vi "Machine_Etat_M1.vi"() -> ()   [LabVIEW 2017]
uses:
  Commande 1.ctl
  enum_tour.ctl
  <vilib>/Platform/TimedLoop/XDataNode/timing_clust.ctl
  <vilib>/Platform/TimedLoop/XDataNode/nitl_modes.ctl
  <vilib>/Platform/TimedLoop/XDataNode/wakeup.ctl
  enum_bras.ctl
  <vilib>/myRIO/Instrument Drivers/Onboard IO/DIO/typedefs/DIO Reference.ctl
  <vilib>/myRIO/Common/Instrument Driver Framework/Utilities/typedefs/myRIO Generic Hardware Reference.ctl
  <vilib>/myRIO/Common/Instrument Driver Framework/Utilities/typedefs/Hardware Version Enum.ctl
  <vilib>/myRIO/Common/Instrument Driver Framework/Utilities/typedefs/myRIO v1.0 Reference.ctl
  <vilib>/myRIO/Common/Instrument Driver Framework/Utilities/typedefs/Generic FPGA Reference.ctl
  <vilib>/myRIO/Common/Instrument Driver Framework/myRIO v1.0/DIO/typedefs/DIO Channels List.ctl
  <vilib>/myRIO/Common/Instrument Driver Framework/myRIO v1.0/DIO/typedefs/DIO Channels Enum.ctl
  <vilib>/userdefined/High Color/nirio_resource_hc.ctl
  <vilib>/myRIO/Common/Instrument Driver Framework/Utilities/vis/Is FPGA Ref Available.vi
  <vilib>/myRIO/Common/Instrument Driver Framework/myRIO v1.0/DIO/vis/myRIO v1.1 Open DIO.vi
  <vilib>/myRIO/Instrument Drivers/Onboard IO/DIO/vis/Write.vi
  <vilib>/myRIO/Common/Instrument Driver Framework/Utilities/vis/Validate Channels.vi
  <vilib>/myRIO/Common/Instrument Driver Framework/myRIO v1.0/DIO/vis/myRIO v1.0 Reserve DIO.vi
  <vilib>/myRIO/Common/Instrument Driver Framework/myRIO v1.0/Resource Manager/vis/myRIO v1.0 Reserve Channel List.vi
  <vilib>/myRIO/Common/Instrument Driver Framework/myRIO v1.0/DIO/vis/myRIO v1.0 Build MUX Configuration DIO.vi
  <vilib>/myRIO/Common/Instrument Driver Framework/myRIO v1.0/Resource Manager/vis/myRIO v1.0 Reserve Channel.vi
  <vilib>/myRIO/Common/Instrument Driver Framework/myRIO v1.0/Resource Manager/vis/myRIO v1.0 Unreserve Channel.vi
  <vilib>/myRIO/Common/Instrument Driver Framework/myRIO v1.0/Resource Manager/vis/myRIO v1.0 Create Configuration List.vi
  <vilib>/myRIO/Common/Instrument Driver Framework/myRIO v1.0/Resource Manager/vis/myRIO v1.0 Build Mutex Name.vi
  <vilib>/Utility/VariantDataType/GetNumericInfo.vi
  <vilib>/Utility/error.llb/Error Cluster From Error Code.vi
  <vilib>/myRIO/Common/Instrument Driver Framework/myRIO v1.0/myRIO v1.1 Open.vi
  <vilib>/myRIO/Common/Instrument Driver Framework/Utilities/vis/IO Manager.vi
  <vilib>/myRIO/Common/Instrument Driver Framework/Utilities/vis/Configuration Manager.vi
  <vilib>/myRIO/Common/Instrument Driver Framework/myRIO v1.0/Resource Manager/vis/myRIO v1.0 Configure IO.vi
  <vilib>/myRIO/Common/Instrument Driver Framework/myRIO v1.0/myRIO v1.0 Close.vi
  <vilib>/myRIO/Common/Instrument Driver Framework/myRIO v1.0/DIO/vis/myRIO v1.0 Write DIO.vi
  <vilib>/Platform/TimedLoop/XDataNode/XDataNode.xnode
  <vilib>/myRIO/Express VI/Onboard Devices/LED/LED Express VI.xnode
  <vilib>/myRIO/Instrument Drivers/Onboard IO/DIO/vis/myRIO DIO Open.xnode
  <vilib>/Platform/TimedLoop/XDataNode/XDNodeRunTimeDep.lvlib
  <vilib>/myRIO/Instrument Drivers/Onboard IO/DIO/DIO.lvlib
panel:
  out "Vert : dévi à droite 2":bool
  out "Graphe déroulant 2":u32(graph)
  out "x > y ? 2":bool[](array[boolean])
  out "Cluster 3":T1
  out "4 LED droite 2":bool[](array[boolean])
  out "4 LED gauche 2":bool[](array[boolean])
  out "droite 2":u32
  out "gauche\n 2":u32
  out "Énum 2":T2
  out "seuil":u32
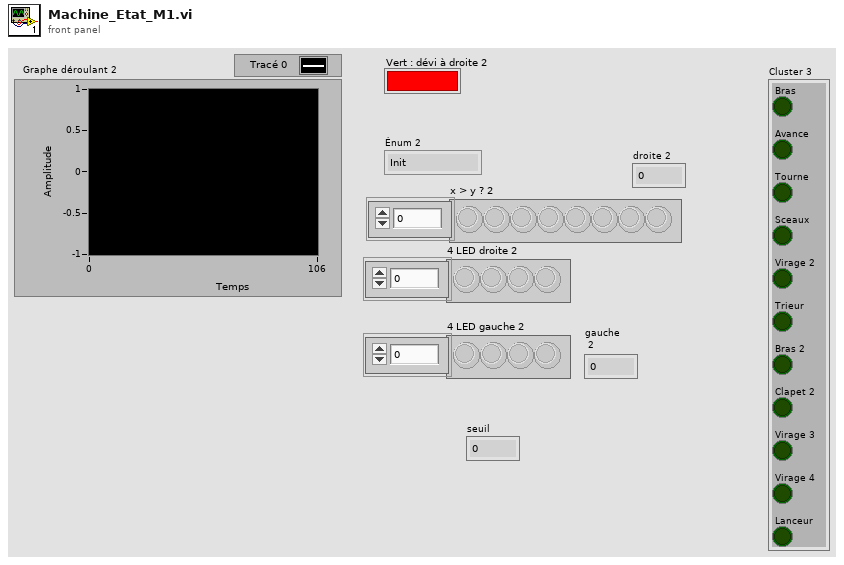
[diagram p1: front panel]
types:
  T1 = typedef "Voyant machine d'état.ctl" = cluster{"Bras":bool, "Avance":bool, "Tourne":bool, "Sceaux":bool, "Virage 2":bool, "Trieur":bool, "Bras 2":bool, "Clapet 2":bool, "Virage 3":bool, "Virage 4":bool, "Lanceur":bool}
  T2 = typedef "Commande 1.ctl" = enum16{"Init", "Bras", "Clapet 1", "Monter_bras", "Virage 1", "Sceaux 0", "Sceaux 1", "Sceaux 2", "Sceaux 3", "Sceaux 4", "Virage 2", "Recule", "Trieur", "Bras 2", "Intersection", "Clapet 2", "Virage 3", "Virage 4", "Avance", "Lanceur", "End", "Monter_bras1", "Monter_bras2", "Avance1", "Avance2", "Intersection1", "Avance3", "Demi_tour", "Virage 5", "Virage 6", "Intersection2", "Intersection3", "Intersection4"}
  T3 = typedef "enum_tour.ctl" = enum16{"Tour1", "Tour2", "Tour3"}
  T4 = typedef "XDNodeRunTimeDep.lvlib/timing_clust.ctl" = cluster{"Expected End [f-1]":u64, "Actual End [f-1]":u64, "Finished Late? [f-1]":bool, "Expected End [i-1]":u64, "Actual End [i-1]":u64, "Finished Late? [i-1]":bool, "Expected Start [i]":u64, "Actual Start [i]":u64, "Expected Start [f]":u64, "Actual Start [f]":u64, "Source Name":string, "Structure Name":string, "Period":i64, "Deadline":i64, "Offset":i64, "Start":i64, "Priority":i32, "Timeout":i32, "Mode":T5, "Wakeup Reason":T6, "Error":errorcluster, "Source Type":string, "Secondary Source Type":string, "Global End Time":u64, "Global Start Time":u64, "Frame Duration":u64, "Iteration Duration":u64, "Assigned CPU":i32, "I/O Scan Engine Mode":u32}
  T5 = typedef "XDNodeRunTimeDep.lvlib/nitl_modes.ctl" = enum32{"No Change", "Process missed periods, maintain original phase", "Discard missed periods, maintain original phase", "Process missed periods, ignore original phase", "Discard missed periods, ignore original phase"}
  T6 = typedef "XDNodeRunTimeDep.lvlib/wakeup.ctl" = enum32{"Normal", "Aborted", "Asynchronous wakeup", "Timing source error", "Timed loop error", "Timeout"}
  T7 = typedef "enum_bras.ctl" = enum16{"Depart Bras", "Clapet Bras", "Inactif Bras", "Seaux Bras"}
  T8 = typedef "DIO.lvlib/DIO Reference.ctl" = cluster{"myRIO Reference":T9, "DIO Channels List":T13}
  T9 = typedef "myRIO Generic Hardware Reference.ctl" = cluster{"myRIO Model":T10, "myRIO Hardware Reference":T11}
  T10 = typedef "Hardware Version Enum.ctl" = enum16{"Unknown", "myRIO-1900", "myRIO-1950", "roboRIO", "NI ELVIS RIO CM"}
  T11 = typedef "myRIO v1.0 Reference.ctl" = cluster{"Generic FPGA Reference":T12, "Allow multiple opens":bool}
  T12 = typedef "Generic FPGA Reference.ctl" = refnum<k20>
  T13 = typedef "DIO Channels List.ctl" = T14[]
  T14 = typedef "DIO Channels Enum.ctl" = enum16{"Not Connected", "C/DIO0", "C/DIO1", "C/DIO2", "C/DIO3", "C/DIO4", "C/DIO5", "C/DIO6", "C/DIO7", "A/DIO0", "A/DIO1", "A/DIO2", "A/DIO3", "A/DIO4", "A/DIO5", "A/DIO6", "A/DIO7", "A/DIO8", "A/DIO9", "A/DIO10", "A/DIO11", "A/DIO12", "A/DIO13", "A/DIO14", "A/DIO15", "B/DIO0", "B/DIO1", "B/DIO2", "B/DIO3", "B/DIO4", "B/DIO5", "B/DIO6", "B/DIO7", "B/DIO8", "B/DIO9", "B/DIO10", "B/DIO11", "B/DIO12", "B/DIO13", "B/DIO14", "B/DIO15", "LED0", "LED1", "LED2", "LED3", "Button0", "DIO/DIO0", "DIO/DIO1", "DIO/DIO2", "DIO/DIO3", "DIO/DIO4", "DIO/DIO5", "DIO/DIO6", "DIO/DIO7", "DIO/DIO8", "DIO/DIO9", "SPI/CS0", "SPI/CS1", "SPI/CS2", "SPI/CS3", "LED RADIO (Green)", "LED RADIO (Red)", "LED COMM (Green)", "LED COMM (Red)", "LED MODE (Green)", "LED MODE (Red)"}
  T15 = typedef "nirio_resource_hc.ctl" = tag
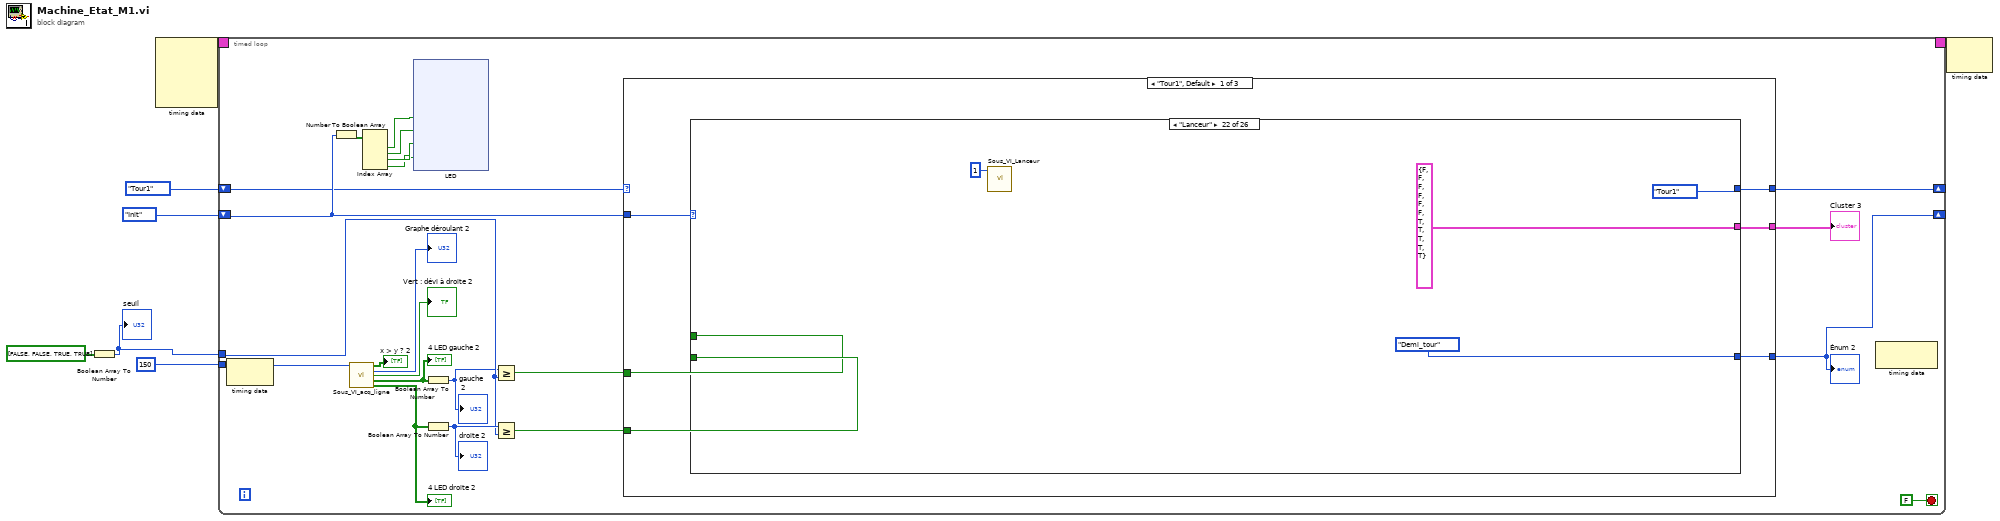
[diagram p0: block diagram]
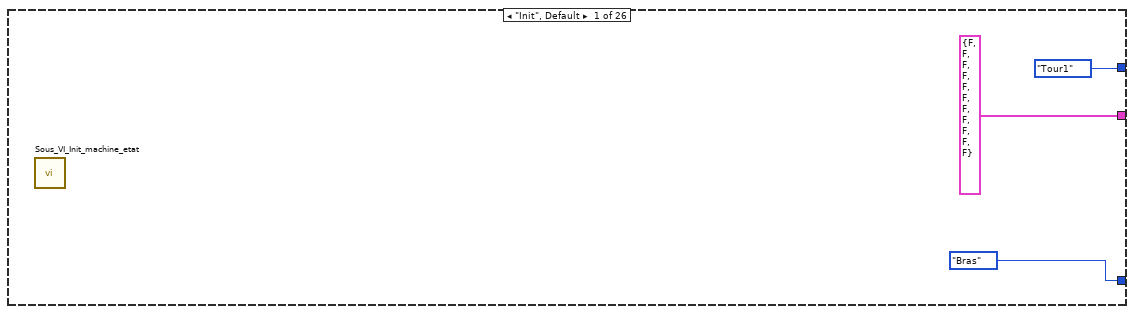
[diagram p2: hidden frame]
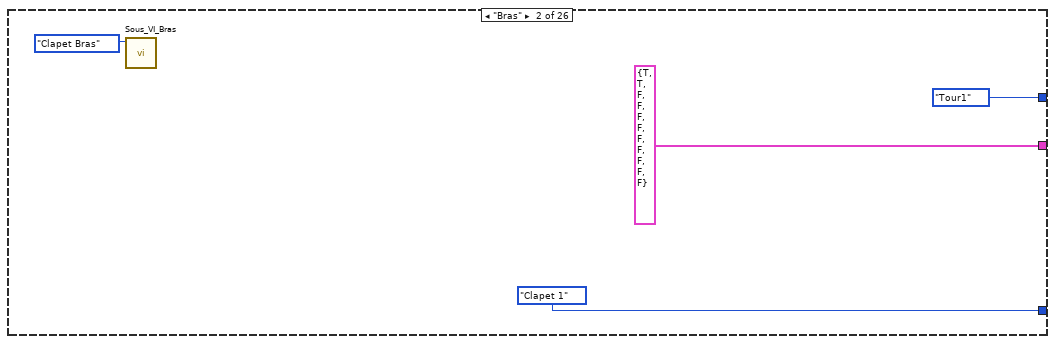
[diagram p3: hidden frame]
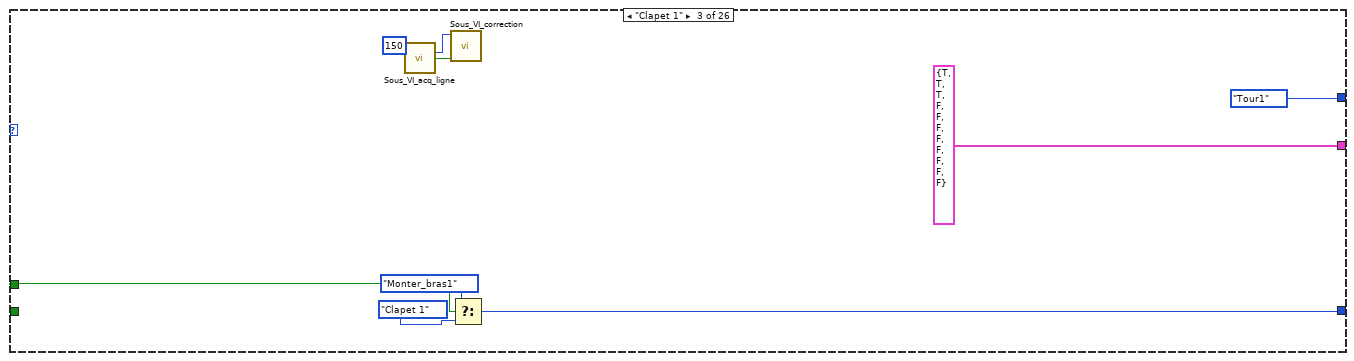
[diagram p4: hidden frame]
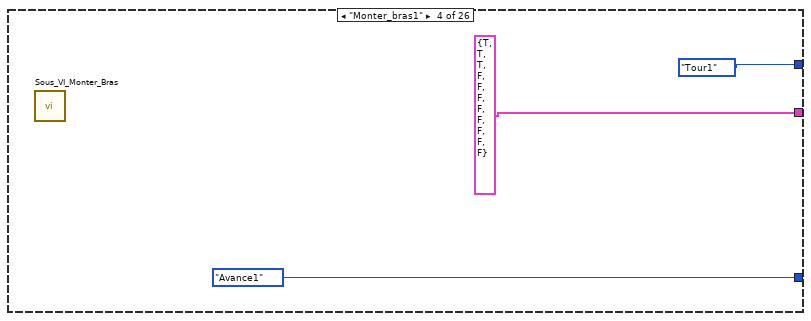
[diagram p5: hidden frame]
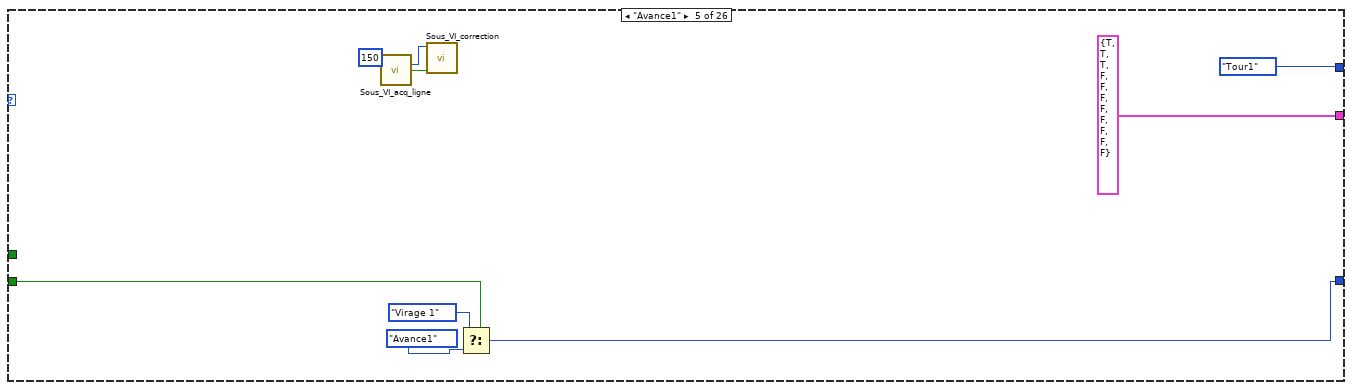
[diagram p6: hidden frame]
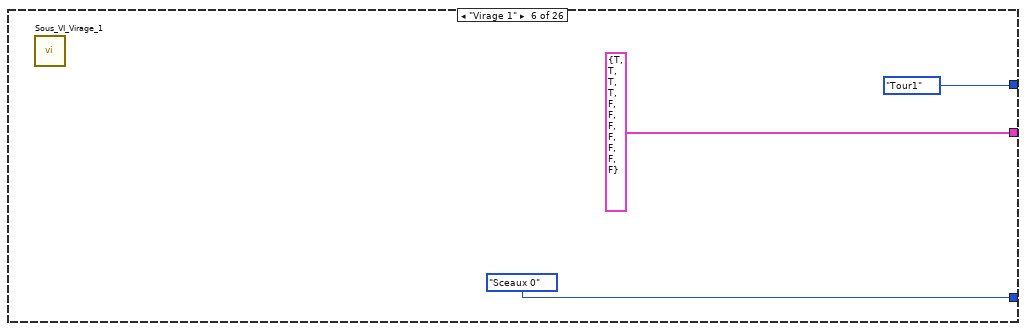
[diagram p7: hidden frame]
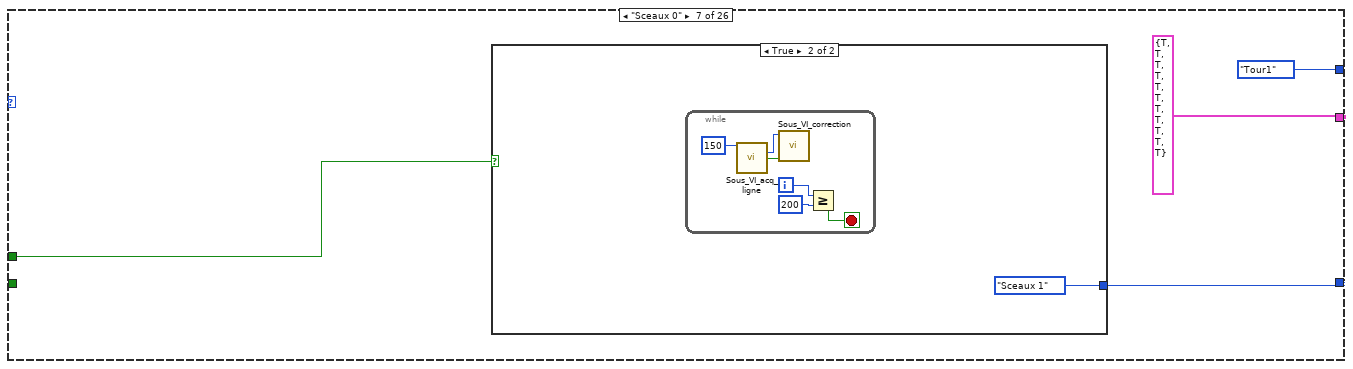
[diagram p8: hidden frame]
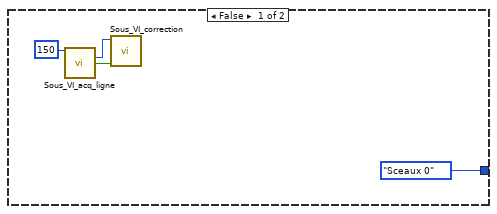
[diagram p9: hidden frame]
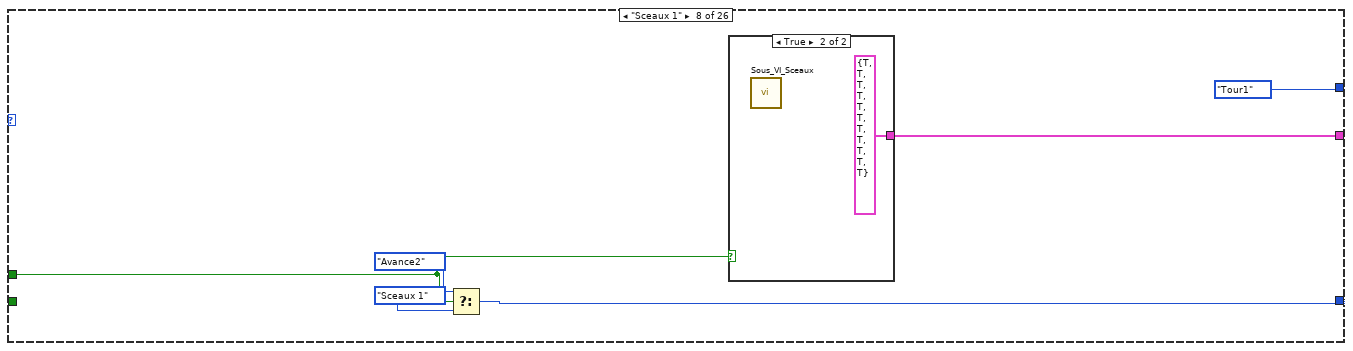
[diagram p10: hidden frame]
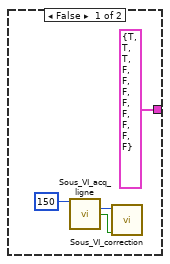
[diagram p11: hidden frame]
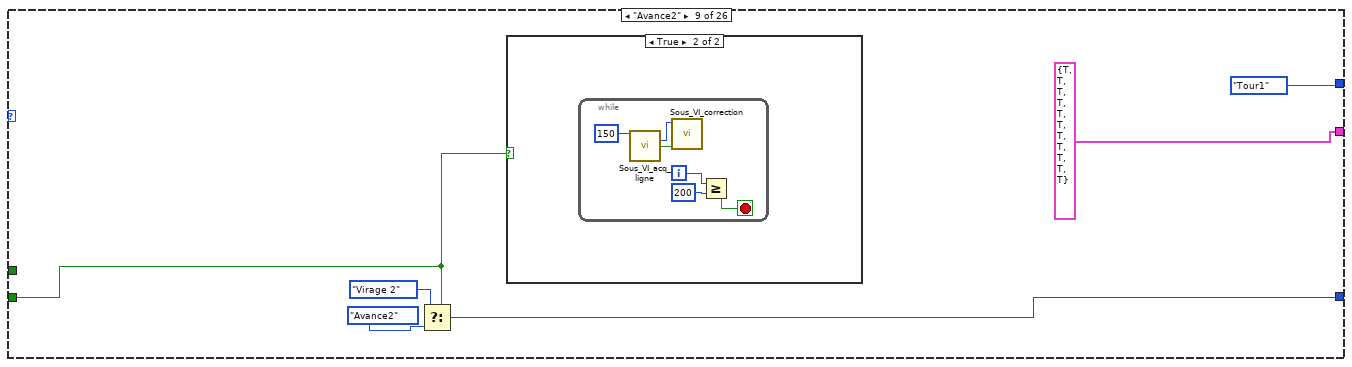
[diagram p12: hidden frame]
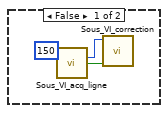
[diagram p13: hidden frame]
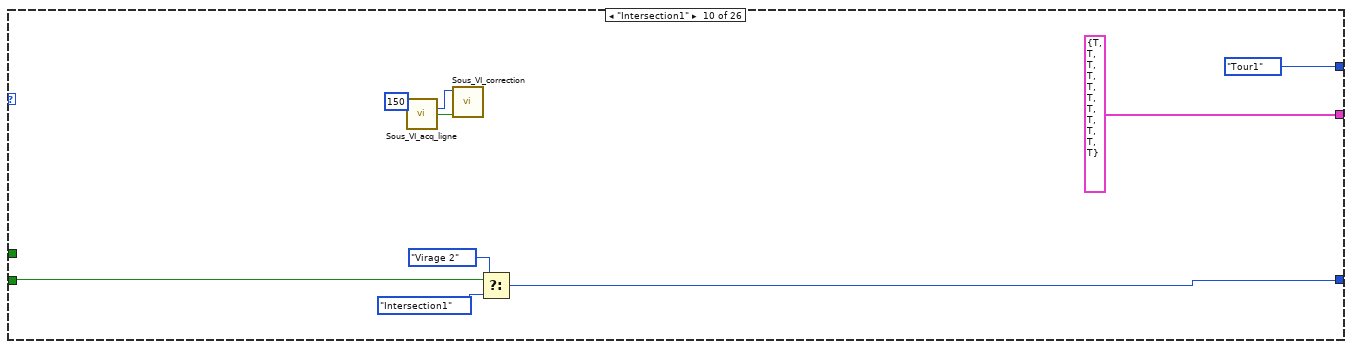
[diagram p14: hidden frame]
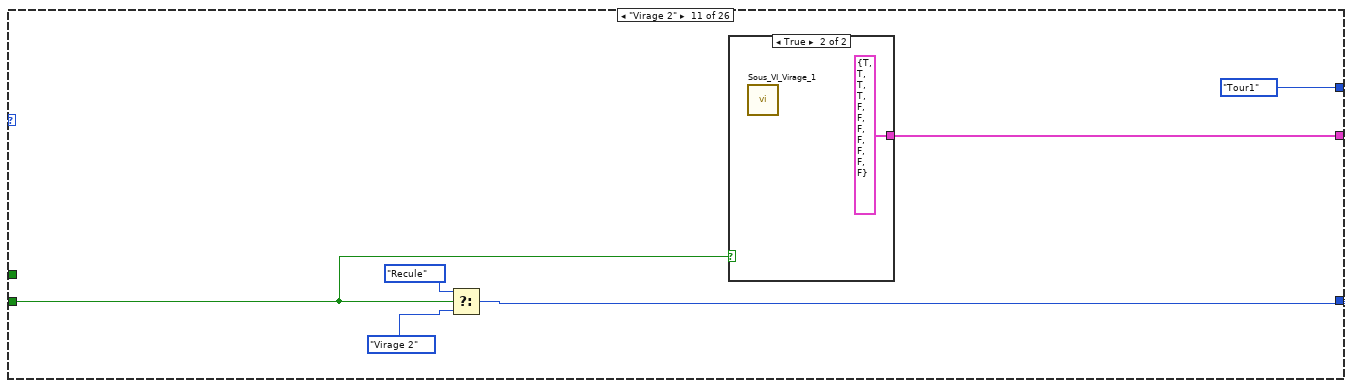
[diagram p15: hidden frame]
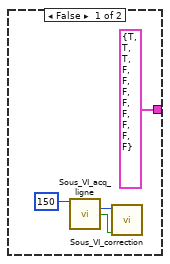
[diagram p16: hidden frame]
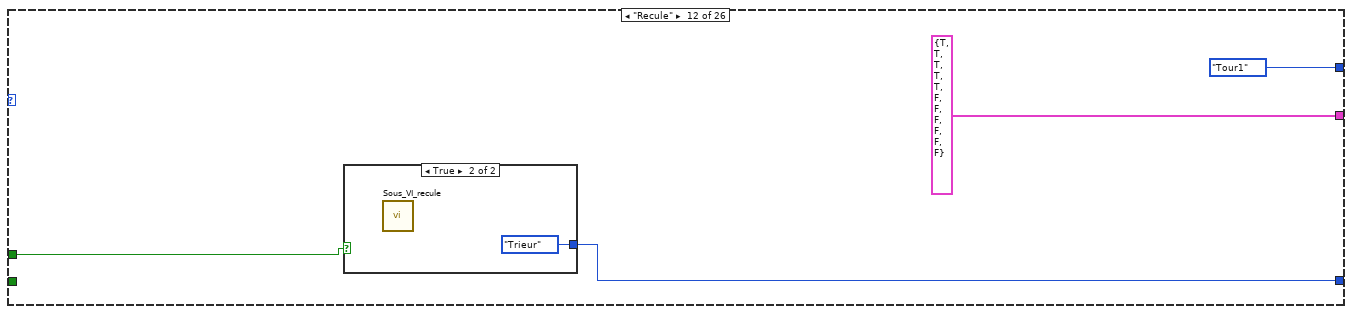
[diagram p17: hidden frame]
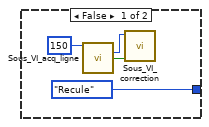
[diagram p18: hidden frame]
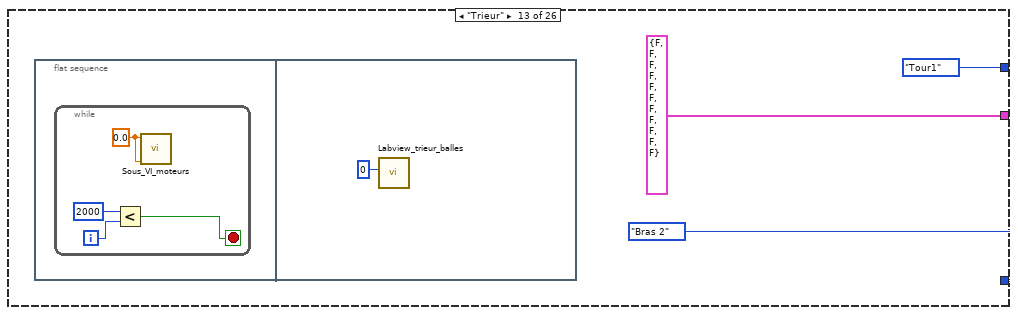
[diagram p19: hidden frame]
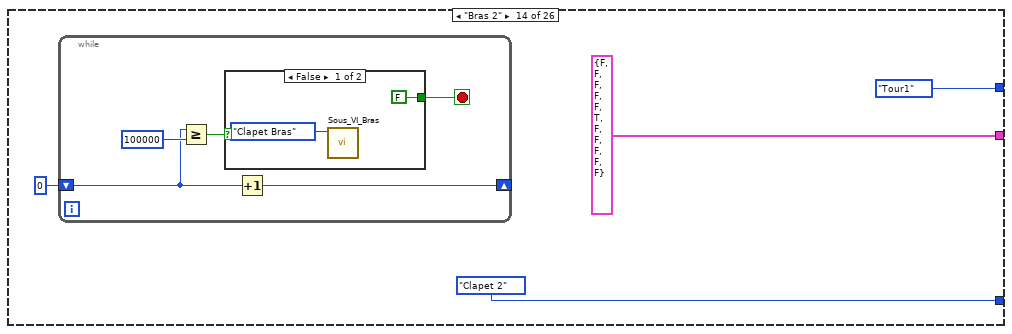
[diagram p20: hidden frame]
diagram:
  n1 = Boolean Array To Number(Boolean array=bool[] [FALSE, FALSE, TRUE, TRUE] ("x < y ? 2")) -> (number=w3:u32)
  "seuil" <- w3
  n2 = node-c288() -> (w6:T4)  [unwired: 4 in]
  n3 = timed-loop {
    tunnel: 150 ("value") -> [w24]
    shift-right: [w29] -> _
    shift-left: Commande_1."Init" -> [w16]
    tunnel: w3 -> [w18]
    timing: w6 -> [_]
    timing-out: [_] -> w5
    shift-right: [w8] -> _
    shift-left: enum_tour."Tour1" -> [w9]
    stop <- FALSE stop-if-true
    n4 = node-c288() -> ()  [unwired: 1 in, 1 out]
    n5 = Number To Boolean Array(number=w16) -> (Boolean array=w15:bool[])
    n6 = call "Sous_VI_acq_ligne.vi"("Seuil"=w24) -> ("x > y ?"=→"x > y ? 2":bool[], "Décalage"=→"Graphe déroulant 2":u32, "G/D ?"=→"Vert : dévi à droite 2":bool, "4 LED gauches"=w21:bool[], "4 LED droite"=w20:bool[])  [unwired: 10 in]
    "4 LED droite 2" <- w20
    "4 LED gauche 2" <- w21
    n7 = Index Array(array=w15) -> (element #1=w14:bool, element #2=w13:bool, element #3=w12:bool, element #4=w11:bool)  [unwired: 4 in]
    n8 = xnode "LED"("LED0"=w14, "LED1"=w13, "LED2"=w12, "LED3"=w11) -> ()  [unwired: 1 in, 1 out]
    n9 = Boolean Array To Number(Boolean array=w21) -> (number=w17:u32)
    "gauche\n 2" <- w17
    n10 = Boolean Array To Number(Boolean array=w20) -> (number=w19:u32)
    "droite 2" <- w19
    n11 = Greater Or Equal?(x=w17, y=w18) -> (x >= y?=w27:bool)
    n12 = Greater Or Equal?(x=w19, y=w18) -> (x >= y?=w28:bool)
    n13 = case shown="\"Tour1\", Default" w9 {
      tunnel: [w35 w234 w469] -> w29
      tunnel: w28 -> [w34 w230 w465]
      tunnel: w27 -> [w33 w231 w466]
      tunnel: [w32 w233 w468] -> w23
      tunnel: w16 -> [w31 w235 w464]
      tunnel: [w30 w232 w467] -> w8
      frame "Tour1", Default {
        n14 = case shown="\"Lanceur\"" w31 {
          tunnel: [Commande_1."Bras" Commande_1."Clapet 1" w49 Commande_1."Avance1" w56 Commande_1."Sceaux 0" w70 w85 w95 w109 w119 w129 Commande_1."Bras 2" Commande_1."Clapet 2" w160 w168 Commande_1."Avance3" w180 Commande_1."Avance" w195 Commande_1."Lanceur" Commande_1."Demi_tour" Commande_1."Virage 5" w212 w220 Commande_1."Intersection2"] -> w35
          tunnel: w34 -> [_ _ _ _ w57 _ _ _ w93 w110 w118 _ _ _ w158 _ _ w179 _ w194 _ _ _ w211 w221 _]
          tunnel: [T1 {"Bras"=FALSE, "Avance"=FALSE, "Tourne"=FALSE, "Sceaux"=FALSE, "Virage 2"=FALSE, "Trieur"=FALSE, "Bras 2"=FALSE, "Clapet 2"=FALSE, "Virage 3"=FALSE, "Virage 4"=FALSE, "Lanceur"=FALSE} ("Cluster 2") T1 {"Bras"=TRUE, "Avance"=TRUE, "Tourne"=FALSE, "Sceaux"=FALSE, "Virage 2"=FALSE, "Trieur"=FALSE, "Bras 2"=FALSE, "Clapet 2"=FALSE, "Virage 3"=FALSE, "Virage 4"=FALSE, "Lanceur"=FALSE} ("Cluster 2") T1 {"Bras"=TRUE, "Avance"=TRUE, "Tourne"=TRUE, "Sceaux"=FALSE, "Virage 2"=FALSE, "Trieur"=FALSE, "Bras 2"=FALSE, "Clapet 2"=FALSE, "Virage 3"=FALSE, "Virage 4"=FALSE, "Lanceur"=FALSE} ("Cluster 2") T1 {"Bras"=TRUE, "Avance"=TRUE, "Tourne"=TRUE, "Sceaux"=FALSE, "Virage 2"=FALSE, "Trieur"=FALSE, "Bras 2"=FALSE, "Clapet 2"=FALSE, "Virage 3"=FALSE, "Virage 4"=FALSE, "Lanceur"=FALSE} ("Cluster 2") T1 {"Bras"=TRUE, "Avance"=TRUE, "Tourne"=TRUE, "Sceaux"=FALSE, "Virage 2"=FALSE, "Trieur"=FALSE, "Bras 2"=FALSE, "Clapet 2"=FALSE, "Virage 3"=FALSE, "Virage 4"=FALSE, "Lanceur"=FALSE} ("Cluster 2") T1 {"Bras"=TRUE, "Avance"=TRUE, "Tourne"=TRUE, "Sceaux"=TRUE, "Virage 2"=FALSE, "Trieur"=FALSE, "Bras 2"=FALSE, "Clapet 2"=FALSE, "Virage 3"=FALSE, "Virage 4"=FALSE, "Lanceur"=FALSE} ("Cluster 2") T1 {"Bras"=TRUE, "Avance"=TRUE, "Tourne"=TRUE, "Sceaux"=TRUE, "Virage 2"=TRUE, "Trieur"=TRUE, "Bras 2"=TRUE, "Clapet 2"=TRUE, "Virage 3"=TRUE, "Virage 4"=TRUE, "Lanceur"=TRUE} ("Cluster 2") w84 T1 {"Bras"=TRUE, "Avance"=TRUE, "Tourne"=TRUE, "Sceaux"=TRUE, "Virage 2"=TRUE, "Trieur"=TRUE, "Bras 2"=TRUE, "Clapet 2"=TRUE, "Virage 3"=TRUE, "Virage 4"=TRUE, "Lanceur"=TRUE} ("Cluster 2") T1 {"Bras"=TRUE, "Avance"=TRUE, "Tourne"=TRUE, "Sceaux"=TRUE, "Virage 2"=TRUE, "Trieur"=TRUE, "Bras 2"=TRUE, "Clapet 2"=TRUE, "Virage 3"=TRUE, "Virage 4"=TRUE, "Lanceur"=TRUE} ("Cluster 2") w122 T1 {"Bras"=TRUE, "Avance"=TRUE, "Tourne"=TRUE, "Sceaux"=TRUE, "Virage 2"=TRUE, "Trieur"=FALSE, "Bras 2"=FALSE, "Clapet 2"=FALSE, "Virage 3"=FALSE, "Virage 4"=FALSE, "Lanceur"=FALSE} ("Cluster 2") T1 {"Bras"=FALSE, "Avance"=FALSE, "Tourne"=FALSE, "Sceaux"=FALSE, "Virage 2"=FALSE, "Trieur"=FALSE, "Bras 2"=FALSE, "Clapet 2"=FALSE, "Virage 3"=FALSE, "Virage 4"=FALSE, "Lanceur"=FALSE} ("Cluster 2") T1 {"Bras"=FALSE, "Avance"=FALSE, "Tourne"=FALSE, "Sceaux"=FALSE, "Virage 2"=FALSE, "Trieur"=TRUE, "Bras 2"=FALSE, "Clapet 2"=FALSE, "Virage 3"=FALSE, "Virage 4"=FALSE, "Lanceur"=FALSE} ("Cluster 2") T1 {"Bras"=FALSE, "Avance"=FALSE, "Tourne"=FALSE, "Sceaux"=FALSE, "Virage 2"=FALSE, "Trieur"=TRUE, "Bras 2"=TRUE, "Clapet 2"=FALSE, "Virage 3"=FALSE, "Virage 4"=FALSE, "Lanceur"=FALSE} ("Cluster 2") T1 {"Bras"=FALSE, "Avance"=FALSE, "Tourne"=FALSE, "Sceaux"=FALSE, "Virage 2"=FALSE, "Trieur"=TRUE, "Bras 2"=TRUE, "Clapet 2"=FALSE, "Virage 3"=FALSE, "Virage 4"=FALSE, "Lanceur"=FALSE} ("Cluster 2") T1 {"Bras"=TRUE, "Avance"=TRUE, "Tourne"=TRUE, "Sceaux"=FALSE, "Virage 2"=FALSE, "Trieur"=FALSE, "Bras 2"=FALSE, "Clapet 2"=FALSE, "Virage 3"=FALSE, "Virage 4"=FALSE, "Lanceur"=FALSE} ("Cluster 2") T1 {"Bras"=TRUE, "Avance"=TRUE, "Tourne"=TRUE, "Sceaux"=TRUE, "Virage 2"=TRUE, "Trieur"=TRUE, "Bras 2"=TRUE, "Clapet 2"=TRUE, "Virage 3"=TRUE, "Virage 4"=TRUE, "Lanceur"=TRUE} ("Cluster 2") T1 {"Bras"=FALSE, "Avance"=FALSE, "Tourne"=FALSE, "Sceaux"=FALSE, "Virage 2"=FALSE, "Trieur"=TRUE, "Bras 2"=TRUE, "Clapet 2"=TRUE, "Virage 3"=TRUE, "Virage 4"=FALSE, "Lanceur"=FALSE} ("Cluster 2") T1 {"Bras"=FALSE, "Avance"=FALSE, "Tourne"=FALSE, "Sceaux"=FALSE, "Virage 2"=FALSE, "Trieur"=FALSE, "Bras 2"=TRUE, "Clapet 2"=TRUE, "Virage 3"=TRUE, "Virage 4"=TRUE, "Lanceur"=FALSE} ("Cluster 2") T1 {"Bras"=FALSE, "Avance"=FALSE, "Tourne"=FALSE, "Sceaux"=FALSE, "Virage 2"=FALSE, "Trieur"=TRUE, "Bras 2"=TRUE, "Clapet 2"=TRUE, "Virage 3"=TRUE, "Virage 4"=TRUE, "Lanceur"=FALSE} ("Cluster 2") T1 {"Bras"=FALSE, "Avance"=FALSE, "Tourne"=FALSE, "Sceaux"=FALSE, "Virage 2"=FALSE, "Trieur"=FALSE, "Bras 2"=TRUE, "Clapet 2"=TRUE, "Virage 3"=TRUE, "Virage 4"=TRUE, "Lanceur"=TRUE} ("Cluster 2") T1 {"Bras"=FALSE, "Avance"=FALSE, "Tourne"=FALSE, "Sceaux"=FALSE, "Virage 2"=FALSE, "Trieur"=TRUE, "Bras 2"=TRUE, "Clapet 2"=TRUE, "Virage 3"=TRUE, "Virage 4"=TRUE, "Lanceur"=FALSE} ("Cluster 2") T1 {"Bras"=FALSE, "Avance"=FALSE, "Tourne"=FALSE, "Sceaux"=FALSE, "Virage 2"=FALSE, "Trieur"=TRUE, "Bras 2"=TRUE, "Clapet 2"=TRUE, "Virage 3"=TRUE, "Virage 4"=TRUE, "Lanceur"=FALSE} ("Cluster 2") T1 {"Bras"=FALSE, "Avance"=FALSE, "Tourne"=FALSE, "Sceaux"=FALSE, "Virage 2"=FALSE, "Trieur"=TRUE, "Bras 2"=TRUE, "Clapet 2"=TRUE, "Virage 3"=TRUE, "Virage 4"=TRUE, "Lanceur"=FALSE} ("Cluster 2") T1 {"Bras"=FALSE, "Avance"=FALSE, "Tourne"=FALSE, "Sceaux"=FALSE, "Virage 2"=FALSE, "Trieur"=FALSE, "Bras 2"=FALSE, "Clapet 2"=FALSE, "Virage 3"=FALSE, "Virage 4"=FALSE, "Lanceur"=FALSE} ("Cluster 2")] -> w32
          tunnel: w33 -> [_ _ w44 _ _ _ w69 w83 _ _ _ w130 _ _ _ w166 _ _ _ _ _ _ _ _ _ _]
          tunnel: [enum_tour."Tour1" enum_tour."Tour1" enum_tour."Tour1" enum_tour."Tour1" enum_tour."Tour1" enum_tour."Tour1" enum_tour."Tour1" enum_tour."Tour1" enum_tour."Tour1" enum_tour."Tour1" enum_tour."Tour1" enum_tour."Tour1" enum_tour."Tour1" enum_tour."Tour1" enum_tour."Tour1" enum_tour."Tour1" enum_tour."Tour1" enum_tour."Tour1" enum_tour."Tour1" enum_tour."Tour1" enum_tour."Tour1" enum_tour."Tour1" enum_tour."Tour1" enum_tour."Tour1" enum_tour."Tour1" enum_tour."Tour2"] -> w30
          frame "Init", Default {
            n15 = call "Sous_VI_Init_machine_etat.vi"() -> ()  [unwired: 12 in]
          }
          frame "Bras" {
            n16 = call "Sous_VI_Bras.vi"("Enum bras"=enum_bras."Clapet Bras") -> ()  [unwired: 11 in]
          }
          frame "Clapet 1" {
            n17 = call "Sous_VI_acq_ligne.vi"("Seuil"=150) -> ("Décalage"=w47:u32, "G/D ?"=w46:bool)  [unwired: 10 in, 3 out]
            n18 = call "Sous_VI_correction.vi"("G/D ?"=w46, "Décalage"=w47) -> ()  [unwired: 10 in]
            n19 = Select(t=Commande_1."Monter_bras1", s=w44, f=Commande_1."Clapet 1") -> (s? t:f=w49:T2)
          }
          frame "Monter_bras1" {
            n20 = call "Sous_VI_Monter_Bras.vi"() -> ()  [unwired: 12 in]
          }
          frame "Avance1" {
            n21 = call "Sous_VI_acq_ligne.vi"("Seuil"=150) -> ("Décalage"=w60:u32, "G/D ?"=w59:bool)  [unwired: 10 in, 3 out]
            n22 = call "Sous_VI_correction.vi"("G/D ?"=w59, "Décalage"=w60) -> ()  [unwired: 10 in]
            n23 = Select(t=Commande_1."Virage 1", s=w57, f=Commande_1."Avance1") -> (s? t:f=w56:T2)
          }
          frame "Virage 1" {
            n24 = call "Sous_VI_Virage_1.vi"() -> ()  [unwired: 12 in]
          }
          frame "Sceaux 0" {
            n25 = case shown="True" w69 {
              tunnel: [Commande_1."Sceaux 0" Commande_1."Sceaux 1"] -> w70
              frame False {
                n26 = call "Sous_VI_acq_ligne.vi"("Seuil"=150) -> ("Décalage"=w73:u32, "G/D ?"=w72:bool)  [unwired: 10 in, 3 out]
                n27 = call "Sous_VI_correction.vi"("G/D ?"=w72, "Décalage"=w73) -> ()  [unwired: 10 in]
              }
              frame True {
                n28 = while {
                  i -> [w81]
                  stop <- w76 stop-if-true
                  n29 = call "Sous_VI_acq_ligne.vi"("Seuil"=150) -> ("Décalage"=w77:u32, "G/D ?"=w78:bool)  [unwired: 10 in, 3 out]
                  n30 = call "Sous_VI_correction.vi"("G/D ?"=w78, "Décalage"=w77) -> ()  [unwired: 10 in]
                  n31 = Greater Or Equal?(x=w81, y=200) -> (x >= y?=w76:bool)
                }
              }
            }
          }
          frame "Sceaux 1" {
            n32 = Select(t=Commande_1."Avance2", s=w83, f=Commande_1."Sceaux 1") -> (s? t:f=w85:T2)
            n33 = case shown="True" w83 {
              tunnel: [T1 {"Bras"=TRUE, "Avance"=TRUE, "Tourne"=TRUE, "Sceaux"=FALSE, "Virage 2"=FALSE, "Trieur"=FALSE, "Bras 2"=FALSE, "Clapet 2"=FALSE, "Virage 3"=FALSE, "Virage 4"=FALSE, "Lanceur"=FALSE} ("Cluster 2") T1 {"Bras"=TRUE, "Avance"=TRUE, "Tourne"=TRUE, "Sceaux"=TRUE, "Virage 2"=TRUE, "Trieur"=TRUE, "Bras 2"=TRUE, "Clapet 2"=TRUE, "Virage 3"=TRUE, "Virage 4"=TRUE, "Lanceur"=TRUE} ("Cluster 2")] -> w84
              frame False {
                n34 = call "Sous_VI_acq_ligne.vi"("Seuil"=150) -> ("Décalage"=w90:u32, "G/D ?"=w89:bool)  [unwired: 10 in, 3 out]
                n35 = call "Sous_VI_correction.vi"("G/D ?"=w89, "Décalage"=w90) -> ()  [unwired: 10 in]
              }
              frame True {
                n36 = call "Sous_VI_Sceaux.vi"() -> ()  [unwired: 12 in]
              }
            }
          }
          frame "Avance2" {
            n37 = Select(t=Commande_1."Virage 2", s=w93, f=Commande_1."Avance2") -> (s? t:f=w95:T2)
            n38 = case shown="True" w93 {
              frame False {
                n39 = call "Sous_VI_acq_ligne.vi"("Seuil"=150) -> ("Décalage"=w99:u32, "G/D ?"=w100:bool)  [unwired: 10 in, 3 out]
                n40 = call "Sous_VI_correction.vi"("G/D ?"=w100, "Décalage"=w99) -> ()  [unwired: 10 in]
              }
              frame True {
                n41 = while {
                  i -> [w107]
                  stop <- w102 stop-if-true
                  n42 = call "Sous_VI_acq_ligne.vi"("Seuil"=150) -> ("Décalage"=w103:u32, "G/D ?"=w104:bool)  [unwired: 10 in, 3 out]
                  n43 = call "Sous_VI_correction.vi"("G/D ?"=w104, "Décalage"=w103) -> ()  [unwired: 10 in]
                  n44 = Greater Or Equal?(x=w107, y=200) -> (x >= y?=w102:bool)
                }
              }
            }
          }
          frame "Intersection1" {
            n45 = call "Sous_VI_acq_ligne.vi"("Seuil"=150) -> ("Décalage"=w114:u32, "G/D ?"=w113:bool)  [unwired: 10 in, 3 out]
            n46 = call "Sous_VI_correction.vi"("G/D ?"=w113, "Décalage"=w114) -> ()  [unwired: 10 in]
            n47 = Select(t=Commande_1."Virage 2", s=w110, f=Commande_1."Intersection1") -> (s? t:f=w109:T2)
          }
          frame "Virage 2" {
            n48 = Select(t=Commande_1."Recule", s=w118, f=Commande_1."Virage 2") -> (s? t:f=w119:T2)
            n49 = case shown="True" w118 {
              tunnel: [T1 {"Bras"=TRUE, "Avance"=TRUE, "Tourne"=TRUE, "Sceaux"=FALSE, "Virage 2"=FALSE, "Trieur"=FALSE, "Bras 2"=FALSE, "Clapet 2"=FALSE, "Virage 3"=FALSE, "Virage 4"=FALSE, "Lanceur"=FALSE} ("Cluster 2") T1 {"Bras"=TRUE, "Avance"=TRUE, "Tourne"=TRUE, "Sceaux"=TRUE, "Virage 2"=FALSE, "Trieur"=FALSE, "Bras 2"=FALSE, "Clapet 2"=FALSE, "Virage 3"=FALSE, "Virage 4"=FALSE, "Lanceur"=FALSE} ("Cluster 2")] -> w122
              frame False {
                n50 = call "Sous_VI_acq_ligne.vi"("Seuil"=150) -> ("Décalage"=w125:u32, "G/D ?"=w124:bool)  [unwired: 10 in, 3 out]
                n51 = call "Sous_VI_correction.vi"("G/D ?"=w124, "Décalage"=w125) -> ()  [unwired: 10 in]
              }
              frame True {
                n52 = call "Sous_VI_Virage_1.vi"() -> ()  [unwired: 12 in]
              }
            }
          }
          frame "Recule" {
            n53 = case shown="True" w130 {
              tunnel: [Commande_1."Recule" Commande_1."Trieur"] -> w129
              frame False {
                n54 = call "Sous_VI_acq_ligne.vi"("Seuil"=150) -> ("Décalage"=w132:u32, "G/D ?"=w135:bool)  [unwired: 10 in, 3 out]
                n55 = call "Sous_VI_correction.vi"("G/D ?"=w135, "Décalage"=w132) -> ()  [unwired: 10 in]
              }
              frame True {
                n56 = call "Sous_VI_recule.vi"() -> ()  [unwired: 12 in]
              }
            }
          }
          frame "Trieur" {
            n57 = flat-sequence {
              frame #0 {
                n58 = while {
                  i -> [w142]
                  stop <- w140 stop-if-true
                  w143 = 0.0 ("moteur gauche vite")
                  n59 = Less?(x=2000, y=w142) -> (x < y?=w140:bool)
                  n60 = call "Sous_VI_moteurs.vi"("Moteur Droit"=w143, "Moteur Gauche"=w143) -> ()  [unwired: 10 in]
                }
              }
              frame #1 {
                n61 = call "Labview_trieur_balles.vi"("Numeric"=0) -> ()  [unwired: 11 in]
              }
            }
          }
          frame "Bras 2" {
            n62 = while {
              shift-right: [w153] -> _
              shift-left: 0 -> [w149]
              stop <- w151 stop-if-true
              n63 = Greater Or Equal?(x=w149, y=100000) -> (x >= y?=w152:bool)
              n64 = case shown="False" w152 {
                tunnel: [FALSE TRUE] -> w151
                frame False {
                  n65 = call "Sous_VI_Bras.vi"("Enum bras"=enum_bras."Clapet Bras") -> ()  [unwired: 11 in]
                }
                frame True {
                }
              }
              n66 = Increment(x=w149) -> (x+1=w153:i32)
            }
          }
          frame "Intersection" {
            n67 = call "Sous_VI_acq_ligne.vi"("Seuil"=150) -> ("Décalage"=w165:u32, "G/D ?"=w164:bool)  [unwired: 10 in, 3 out]
            n68 = call "Sous_VI_correction.vi"("G/D ?"=w164, "Décalage"=w165) -> ()  [unwired: 10 in]
            n69 = Select(t=Commande_1."Clapet 2", s=w158, f=Commande_1."Intersection") -> (s? t:f=w160:T2)
          }
          frame "Clapet 2" {
            n70 = call "Sous_VI_acq_ligne.vi"("Seuil"=150) -> ("Décalage"=w173:u32, "G/D ?"=w172:bool)  [unwired: 10 in, 3 out]
            n71 = call "Sous_VI_correction.vi"("G/D ?"=w172, "Décalage"=w173) -> ()  [unwired: 10 in]
            n72 = Select(t=Commande_1."Monter_bras2", s=w166, f=Commande_1."Clapet 2") -> (s? t:f=w168:T2)
          }
          frame "Monter_bras2" {
            n73 = call "Sous_VI_Monter_Bras.vi"() -> ()  [unwired: 12 in]
          }
          frame "Avance3" {
            n74 = call "Sous_VI_acq_ligne.vi"("Seuil"=150) -> ("Décalage"=w184:u32, "G/D ?"=w183:bool)  [unwired: 10 in, 3 out]
            n75 = call "Sous_VI_correction.vi"("G/D ?"=w183, "Décalage"=w184) -> ()  [unwired: 10 in]
            n76 = Select(t=Commande_1."Virage 3", s=w179, f=Commande_1."Avance3") -> (s? t:f=w180:T2)
          }
          frame "Virage 3" {
            n77 = call "Sous_VI_Virage_1.vi"() -> ()  [unwired: 12 in]
          }
          frame "Avance" {
            n78 = call "Sous_VI_acq_ligne.vi"("Seuil"=150) -> ("Décalage"=w193:u32, "G/D ?"=w192:bool)  [unwired: 10 in, 3 out]
            n79 = call "Sous_VI_correction.vi"("G/D ?"=w192, "Décalage"=w193) -> ()  [unwired: 10 in]
            n80 = Select(t=Commande_1."Virage 4", s=w194, f=Commande_1."Avance") -> (s? t:f=w195:T2)
          }
          frame "Virage 4" {
            n81 = call "Sous_VI_Virage_1.vi"() -> ()  [unwired: 12 in]
          }
          frame "Lanceur" {
            n82 = call "Sous_VI_Lanceur.vi"("Nb balles"=1) -> ()  [unwired: 11 in]
          }
          frame "Demi_tour" {
            n83 = call "Sous_VI_Virage_1.vi"() -> ()  [unwired: 12 in]
          }
          frame "Virage 5" {
            n84 = case shown="True" w211 {
              tunnel: [Commande_1."Virage 5" Commande_1."Virage 6"] -> w212
              frame False {
                n85 = call "Sous_VI_acq_ligne.vi"("Seuil"=150) -> ("Décalage"=w216:u32, "G/D ?"=w215:bool)  [unwired: 10 in, 3 out]
                n86 = call "Sous_VI_correction.vi"("G/D ?"=w215, "Décalage"=w216) -> ()  [unwired: 10 in]
              }
              frame True {
                n87 = call "Sous_VI_Virage_cible.vi"() -> ()  [unwired: 12 in]
              }
            }
          }
          frame "Virage 6" {
            n88 = case shown="True" w221 {
              tunnel: [Commande_1."Virage 6" Commande_1."End"] -> w220
              frame False {
                n89 = call "Sous_VI_acq_ligne.vi"("Seuil"=150) -> ("Décalage"=w225:u32, "G/D ?"=w224:bool)  [unwired: 10 in, 3 out]
                n90 = call "Sous_VI_correction.vi"("G/D ?"=w224, "Décalage"=w225) -> ()  [unwired: 10 in]
              }
              frame True {
                n91 = call "Sous_VI_Virage_1.vi"() -> ()  [unwired: 12 in]
              }
            }
          }
          frame "End" {
          }
        }
      }
      frame "Tour2" {
        n92 = case shown="\"Intersection2\", Default" w235 {
          tunnel: [w240 Commande_1."Clapet 1" w268 Commande_1."Avance1" w275 Commande_1."Sceaux 0" w289 w307 w323 w333 w343 w353 Commande_1."Intersection" w372 Commande_1."Clapet 2" w402 Commande_1."Avance3" w414 Commande_1."Avance" w429 Commande_1."Lanceur" Commande_1."Demi_tour" Commande_1."Virage 5" w446 w454 Commande_1."Intersection2"] -> w234
          tunnel: w230 -> [_ _ _ _ w276 _ _ _ _ w334 w342 _ _ _ _ _ _ w413 _ w428 _ _ _ w445 w455 _]
          tunnel: [T1 {"Bras"=TRUE, "Avance"=TRUE, "Tourne"=FALSE, "Sceaux"=FALSE, "Virage 2"=FALSE, "Trieur"=FALSE, "Bras 2"=FALSE, "Clapet 2"=FALSE, "Virage 3"=FALSE, "Virage 4"=FALSE, "Lanceur"=FALSE} ("Cluster 2") T1 {"Bras"=TRUE, "Avance"=TRUE, "Tourne"=FALSE, "Sceaux"=FALSE, "Virage 2"=FALSE, "Trieur"=FALSE, "Bras 2"=FALSE, "Clapet 2"=FALSE, "Virage 3"=FALSE, "Virage 4"=FALSE, "Lanceur"=FALSE} ("Cluster 2") T1 {"Bras"=TRUE, "Avance"=TRUE, "Tourne"=TRUE, "Sceaux"=FALSE, "Virage 2"=FALSE, "Trieur"=FALSE, "Bras 2"=FALSE, "Clapet 2"=FALSE, "Virage 3"=FALSE, "Virage 4"=FALSE, "Lanceur"=FALSE} ("Cluster 2") T1 {"Bras"=TRUE, "Avance"=TRUE, "Tourne"=TRUE, "Sceaux"=FALSE, "Virage 2"=FALSE, "Trieur"=FALSE, "Bras 2"=FALSE, "Clapet 2"=FALSE, "Virage 3"=FALSE, "Virage 4"=FALSE, "Lanceur"=FALSE} ("Cluster 2") T1 {"Bras"=TRUE, "Avance"=TRUE, "Tourne"=TRUE, "Sceaux"=FALSE, "Virage 2"=FALSE, "Trieur"=FALSE, "Bras 2"=FALSE, "Clapet 2"=FALSE, "Virage 3"=FALSE, "Virage 4"=FALSE, "Lanceur"=FALSE} ("Cluster 2") T1 {"Bras"=TRUE, "Avance"=TRUE, "Tourne"=TRUE, "Sceaux"=TRUE, "Virage 2"=FALSE, "Trieur"=FALSE, "Bras 2"=FALSE, "Clapet 2"=FALSE, "Virage 3"=FALSE, "Virage 4"=FALSE, "Lanceur"=FALSE} ("Cluster 2") T1 {"Bras"=TRUE, "Avance"=TRUE, "Tourne"=TRUE, "Sceaux"=TRUE, "Virage 2"=TRUE, "Trieur"=TRUE, "Bras 2"=TRUE, "Clapet 2"=TRUE, "Virage 3"=TRUE, "Virage 4"=TRUE, "Lanceur"=TRUE} ("Cluster 2") w306 w322 T1 {"Bras"=TRUE, "Avance"=TRUE, "Tourne"=TRUE, "Sceaux"=TRUE, "Virage 2"=TRUE, "Trieur"=TRUE, "Bras 2"=TRUE, "Clapet 2"=TRUE, "Virage 3"=TRUE, "Virage 4"=TRUE, "Lanceur"=TRUE} ("Cluster 2") w346 T1 {"Bras"=TRUE, "Avance"=TRUE, "Tourne"=TRUE, "Sceaux"=TRUE, "Virage 2"=TRUE, "Trieur"=FALSE, "Bras 2"=FALSE, "Clapet 2"=FALSE, "Virage 3"=FALSE, "Virage 4"=FALSE, "Lanceur"=FALSE} ("Cluster 2") T1 {"Bras"=FALSE, "Avance"=FALSE, "Tourne"=FALSE, "Sceaux"=FALSE, "Virage 2"=FALSE, "Trieur"=FALSE, "Bras 2"=FALSE, "Clapet 2"=FALSE, "Virage 3"=FALSE, "Virage 4"=FALSE, "Lanceur"=FALSE} ("Cluster 2") T1 {"Bras"=FALSE, "Avance"=FALSE, "Tourne"=FALSE, "Sceaux"=FALSE, "Virage 2"=FALSE, "Trieur"=TRUE, "Bras 2"=TRUE, "Clapet 2"=FALSE, "Virage 3"=FALSE, "Virage 4"=FALSE, "Lanceur"=FALSE} ("Cluster 2") T1 {"Bras"=FALSE, "Avance"=FALSE, "Tourne"=FALSE, "Sceaux"=FALSE, "Virage 2"=FALSE, "Trieur"=TRUE, "Bras 2"=FALSE, "Clapet 2"=FALSE, "Virage 3"=FALSE, "Virage 4"=FALSE, "Lanceur"=FALSE} ("Cluster 2") T1 {"Bras"=FALSE, "Avance"=FALSE, "Tourne"=FALSE, "Sceaux"=FALSE, "Virage 2"=FALSE, "Trieur"=TRUE, "Bras 2"=TRUE, "Clapet 2"=FALSE, "Virage 3"=FALSE, "Virage 4"=FALSE, "Lanceur"=FALSE} ("Cluster 2") T1 {"Bras"=TRUE, "Avance"=TRUE, "Tourne"=TRUE, "Sceaux"=FALSE, "Virage 2"=FALSE, "Trieur"=FALSE, "Bras 2"=FALSE, "Clapet 2"=FALSE, "Virage 3"=FALSE, "Virage 4"=FALSE, "Lanceur"=FALSE} ("Cluster 2") T1 {"Bras"=TRUE, "Avance"=TRUE, "Tourne"=TRUE, "Sceaux"=TRUE, "Virage 2"=TRUE, "Trieur"=TRUE, "Bras 2"=TRUE, "Clapet 2"=TRUE, "Virage 3"=TRUE, "Virage 4"=TRUE, "Lanceur"=TRUE} ("Cluster 2") T1 {"Bras"=FALSE, "Avance"=FALSE, "Tourne"=FALSE, "Sceaux"=FALSE, "Virage 2"=FALSE, "Trieur"=TRUE, "Bras 2"=TRUE, "Clapet 2"=TRUE, "Virage 3"=TRUE, "Virage 4"=FALSE, "Lanceur"=FALSE} ("Cluster 2") T1 {"Bras"=FALSE, "Avance"=FALSE, "Tourne"=FALSE, "Sceaux"=FALSE, "Virage 2"=FALSE, "Trieur"=FALSE, "Bras 2"=TRUE, "Clapet 2"=TRUE, "Virage 3"=TRUE, "Virage 4"=TRUE, "Lanceur"=FALSE} ("Cluster 2") T1 {"Bras"=FALSE, "Avance"=FALSE, "Tourne"=FALSE, "Sceaux"=FALSE, "Virage 2"=FALSE, "Trieur"=TRUE, "Bras 2"=TRUE, "Clapet 2"=TRUE, "Virage 3"=TRUE, "Virage 4"=TRUE, "Lanceur"=FALSE} ("Cluster 2") T1 {"Bras"=FALSE, "Avance"=FALSE, "Tourne"=FALSE, "Sceaux"=FALSE, "Virage 2"=FALSE, "Trieur"=FALSE, "Bras 2"=TRUE, "Clapet 2"=TRUE, "Virage 3"=TRUE, "Virage 4"=TRUE, "Lanceur"=TRUE} ("Cluster 2") T1 {"Bras"=FALSE, "Avance"=FALSE, "Tourne"=FALSE, "Sceaux"=FALSE, "Virage 2"=FALSE, "Trieur"=TRUE, "Bras 2"=TRUE, "Clapet 2"=TRUE, "Virage 3"=TRUE, "Virage 4"=TRUE, "Lanceur"=FALSE} ("Cluster 2") T1 {"Bras"=FALSE, "Avance"=FALSE, "Tourne"=FALSE, "Sceaux"=FALSE, "Virage 2"=FALSE, "Trieur"=TRUE, "Bras 2"=TRUE, "Clapet 2"=TRUE, "Virage 3"=TRUE, "Virage 4"=TRUE, "Lanceur"=FALSE} ("Cluster 2") T1 {"Bras"=FALSE, "Avance"=FALSE, "Tourne"=FALSE, "Sceaux"=FALSE, "Virage 2"=FALSE, "Trieur"=TRUE, "Bras 2"=TRUE, "Clapet 2"=TRUE, "Virage 3"=TRUE, "Virage 4"=TRUE, "Lanceur"=FALSE} ("Cluster 2") T1 {"Bras"=FALSE, "Avance"=FALSE, "Tourne"=FALSE, "Sceaux"=FALSE, "Virage 2"=FALSE, "Trieur"=FALSE, "Bras 2"=FALSE, "Clapet 2"=FALSE, "Virage 3"=FALSE, "Virage 4"=FALSE, "Lanceur"=FALSE} ("Cluster 2")] -> w233
          tunnel: w231 -> [w239 _ w263 _ _ _ w288 w305 w324 _ _ w354 _ w369 _ w400 _ _ _ _ _ _ _ _ _ _]
          tunnel: [enum_tour."Tour2" enum_tour."Tour2" enum_tour."Tour2" enum_tour."Tour2" enum_tour."Tour2" enum_tour."Tour2" enum_tour."Tour2" enum_tour."Tour2" enum_tour."Tour2" enum_tour."Tour2" enum_tour."Tour2" enum_tour."Tour2" enum_tour."Tour2" enum_tour."Tour2" enum_tour."Tour2" enum_tour."Tour2" enum_tour."Tour2" enum_tour."Tour2" enum_tour."Tour2" enum_tour."Tour2" enum_tour."Tour2" enum_tour."Tour2" enum_tour."Tour2" enum_tour."Tour2" enum_tour."Tour2" enum_tour."Tour3"] -> w232
          frame "Intersection2", Default {
            n93 = call "Sous_VI_acq_ligne.vi"("Seuil"=150) -> ("Décalage"=w238:u32, "G/D ?"=w237:bool)  [unwired: 10 in, 3 out]
            n94 = call "Sous_VI_correction.vi"("G/D ?"=w237, "Décalage"=w238) -> ()  [unwired: 10 in]
            n95 = Select(t=Commande_1."Bras", s=w239, f=Commande_1."Intersection2") -> (s? t:f=w240:T2)
          }
          frame "Bras" {
            n96 = flat-sequence {
              frame #0 {
                n97 = while {
                  i -> [w253]
                  stop <- w251 stop-if-true
                  n98 = Less?(x=1500, y=w253) -> (x < y?=w251:bool)
                  n99 = call "Sous_VI_acq_ligne.vi"("Seuil"=150) -> ("Décalage"=w249:u32, "G/D ?"=w248:bool)  [unwired: 10 in, 3 out]
                  n100 = call "Sous_VI_correction.vi"("G/D ?"=w248, "Décalage"=w249) -> ()  [unwired: 10 in]
                }
              }
              frame #1 {
                n101 = while {
                  i -> [w257]
                  stop <- w255 stop-if-true
                  w254 = 0.0 ("moteur gauche vite")
                  n102 = Less?(x=1500, y=w257) -> (x < y?=w255:bool)
                  n103 = call "Sous_VI_moteurs.vi"("Moteur Droit"=w254, "Moteur Gauche"=w254) -> ()  [unwired: 10 in]
                }
              }
              frame #2 {
                n104 = while {
                  i -> [w261]
                  stop <- w259 stop-if-true
                  n105 = Less?(x=1500, y=w261) -> (x < y?=w259:bool)
                  n106 = call "Sous_VI_Bras.vi"("Enum bras"=enum_bras."Clapet Bras") -> ()  [unwired: 11 in]
                }
              }
            }
          }
          frame "Clapet 1" {
            n107 = call "Sous_VI_acq_ligne.vi"("Seuil"=150) -> ("Décalage"=w266:u32, "G/D ?"=w265:bool)  [unwired: 10 in, 3 out]
            n108 = call "Sous_VI_correction.vi"("G/D ?"=w265, "Décalage"=w266) -> ()  [unwired: 10 in]
            n109 = Select(t=Commande_1."Monter_bras1", s=w263, f=Commande_1."Clapet 1") -> (s? t:f=w268:T2)
          }
          frame "Monter_bras1" {
            n110 = call "Sous_VI_Monter_Bras.vi"() -> ()  [unwired: 12 in]
          }
          frame "Avance1" {
            n111 = call "Sous_VI_acq_ligne.vi"("Seuil"=150) -> ("Décalage"=w279:u32, "G/D ?"=w278:bool)  [unwired: 10 in, 3 out]
            n112 = call "Sous_VI_correction.vi"("G/D ?"=w278, "Décalage"=w279) -> ()  [unwired: 10 in]
            n113 = Select(t=Commande_1."Virage 1", s=w276, f=Commande_1."Avance1") -> (s? t:f=w275:T2)
          }
          frame "Virage 1" {
            n114 = call "Sous_VI_Virage_1.vi"() -> ()  [unwired: 12 in]
          }
          frame "Sceaux 0" {
            n115 = case shown="True" w288 {
              tunnel: [Commande_1."Sceaux 0" Commande_1."Sceaux 1"] -> w289
              frame False {
                n116 = call "Sous_VI_acq_ligne.vi"("Seuil"=150) -> ("Décalage"=w292:u32, "G/D ?"=w291:bool)  [unwired: 10 in, 3 out]
                n117 = call "Sous_VI_correction.vi"("G/D ?"=w291, "Décalage"=w292) -> ()  [unwired: 10 in]
              }
              frame True {
                n118 = while {
                  i -> [w298]
                  stop <- w295 stop-if-true
                  n119 = Greater Or Equal?(x=w298, y=200) -> (x >= y?=w296:bool)
                  n120 = case shown="False" w296 {
                    tunnel: [FALSE TRUE] -> w295
                    frame False {
                      n121 = call "Sous_VI_acq_ligne.vi"("Seuil"=150) -> ("Décalage"=w302:u32, "G/D ?"=w301:bool)  [unwired: 10 in, 3 out]
                      n122 = call "Sous_VI_correction.vi"("G/D ?"=w301, "Décalage"=w302) -> ()  [unwired: 10 in]
                    }
                    frame True {
                    }
                  }
                }
              }
            }
          }
          frame "Sceaux 1" {
            n123 = Select(t=Commande_1."Sceaux 2", s=w305, f=Commande_1."Sceaux 1") -> (s? t:f=w307:T2)
            n124 = case shown="True" w305 {
              tunnel: [T1 {"Bras"=TRUE, "Avance"=TRUE, "Tourne"=TRUE, "Sceaux"=FALSE, "Virage 2"=FALSE, "Trieur"=FALSE, "Bras 2"=FALSE, "Clapet 2"=FALSE, "Virage 3"=FALSE, "Virage 4"=FALSE, "Lanceur"=FALSE} ("Cluster 2") T1 {"Bras"=TRUE, "Avance"=TRUE, "Tourne"=TRUE, "Sceaux"=TRUE, "Virage 2"=TRUE, "Trieur"=TRUE, "Bras 2"=TRUE, "Clapet 2"=TRUE, "Virage 3"=TRUE, "Virage 4"=TRUE, "Lanceur"=TRUE} ("Cluster 2")] -> w306
              frame False {
                n125 = call "Sous_VI_acq_ligne.vi"("Seuil"=150) -> ("Décalage"=w312:u32, "G/D ?"=w311:bool)  [unwired: 10 in, 3 out]
                n126 = call "Sous_VI_correction.vi"("G/D ?"=w311, "Décalage"=w312) -> ()  [unwired: 10 in]
              }
              frame True {
                n127 = while {
                  i -> [w320]
                  stop <- w315 stop-if-true
                  n128 = call "Sous_VI_acq_ligne.vi"("Seuil"=150) -> ("Décalage"=w316:u32, "G/D ?"=w317:bool)  [unwired: 10 in, 3 out]
                  n129 = call "Sous_VI_correction.vi"("G/D ?"=w317, "Décalage"=w316) -> ()  [unwired: 10 in]
                  n130 = Greater Or Equal?(x=w320, y=200) -> (x >= y?=w315:bool)
                }
              }
            }
          }
          frame "Sceaux 2" {
            n131 = Select(t=Commande_1."Virage 2", s=w324, f=Commande_1."Sceaux 2") -> (s? t:f=w323:T2)
            n132 = case shown="True" w324 {
              tunnel: [T1 {"Bras"=TRUE, "Avance"=TRUE, "Tourne"=TRUE, "Sceaux"=FALSE, "Virage 2"=FALSE, "Trieur"=FALSE, "Bras 2"=FALSE, "Clapet 2"=FALSE, "Virage 3"=FALSE, "Virage 4"=FALSE, "Lanceur"=FALSE} ("Cluster 2") T1 {"Bras"=TRUE, "Avance"=TRUE, "Tourne"=TRUE, "Sceaux"=TRUE, "Virage 2"=TRUE, "Trieur"=TRUE, "Bras 2"=TRUE, "Clapet 2"=TRUE, "Virage 3"=TRUE, "Virage 4"=TRUE, "Lanceur"=TRUE} ("Cluster 2")] -> w322
              frame False {
                n133 = call "Sous_VI_acq_ligne.vi"("Seuil"=150) -> ("Décalage"=w329:u32, "G/D ?"=w328:bool)  [unwired: 10 in, 3 out]
                n134 = call "Sous_VI_correction.vi"("G/D ?"=w328, "Décalage"=w329) -> ()  [unwired: 10 in]
              }
              frame True {
                n135 = call "Sous_VI_Sceaux.vi"() -> ()  [unwired: 12 in]
              }
            }
          }
          frame "Avance2" {
            n136 = call "Sous_VI_acq_ligne.vi"("Seuil"=150) -> ("Décalage"=w337:u32, "G/D ?"=w336:bool)  [unwired: 10 in, 3 out]
            n137 = call "Sous_VI_correction.vi"("G/D ?"=w336, "Décalage"=w337) -> ()  [unwired: 10 in]
            n138 = Select(t=Commande_1."Virage 2", s=w334, f=Commande_1."Avance2") -> (s? t:f=w333:T2)
          }
          frame "Virage 2" {
            n139 = Select(t=Commande_1."Recule", s=w342, f=Commande_1."Virage 2") -> (s? t:f=w343:T2)
            n140 = case shown="True" w342 {
              tunnel: [T1 {"Bras"=TRUE, "Avance"=TRUE, "Tourne"=TRUE, "Sceaux"=FALSE, "Virage 2"=FALSE, "Trieur"=FALSE, "Bras 2"=FALSE, "Clapet 2"=FALSE, "Virage 3"=FALSE, "Virage 4"=FALSE, "Lanceur"=FALSE} ("Cluster 2") T1 {"Bras"=TRUE, "Avance"=TRUE, "Tourne"=TRUE, "Sceaux"=TRUE, "Virage 2"=FALSE, "Trieur"=FALSE, "Bras 2"=FALSE, "Clapet 2"=FALSE, "Virage 3"=FALSE, "Virage 4"=FALSE, "Lanceur"=FALSE} ("Cluster 2")] -> w346
              frame False {
                n141 = call "Sous_VI_acq_ligne.vi"("Seuil"=150) -> ("Décalage"=w349:u32, "G/D ?"=w348:bool)  [unwired: 10 in, 3 out]
                n142 = call "Sous_VI_correction.vi"("G/D ?"=w348, "Décalage"=w349) -> ()  [unwired: 10 in]
              }
              frame True {
                n143 = call "Sous_VI_Virage_1.vi"() -> ()  [unwired: 12 in]
              }
            }
          }
          frame "Recule" {
            n144 = case shown="True" w354 {
              tunnel: [Commande_1."Recule" Commande_1."Trieur"] -> w353
              frame False {
                n145 = call "Sous_VI_acq_ligne.vi"("Seuil"=150) -> ("Décalage"=w356:u32, "G/D ?"=w359:bool)  [unwired: 10 in, 3 out]
                n146 = call "Sous_VI_correction.vi"("G/D ?"=w359, "Décalage"=w356) -> ()  [unwired: 10 in]
              }
              frame True {
                n147 = call "Sous_VI_recule.vi"() -> ()  [unwired: 12 in]
              }
            }
          }
          frame "Trieur" {
            n148 = flat-sequence {
              frame #0 {
                n149 = while {
                  i -> [w366]
                  stop <- w364 stop-if-true
                  w367 = 0.0 ("moteur gauche vite")
                  n150 = Less?(x=2000, y=w366) -> (x < y?=w364:bool)
                  n151 = call "Sous_VI_moteurs.vi"("Moteur Droit"=w367, "Moteur Gauche"=w367) -> ()  [unwired: 10 in]
                }
              }
              frame #1 {
                n152 = call "Labview_trieur_balles.vi"("Numeric"=2) -> ()  [unwired: 11 in]
              }
            }
          }
          frame "Intersection" {
            n153 = call "Sous_VI_acq_ligne.vi"("Seuil"=150) -> ("Décalage"=w377:u32, "G/D ?"=w376:bool)  [unwired: 10 in, 3 out]
            n154 = call "Sous_VI_correction.vi"("G/D ?"=w376, "Décalage"=w377) -> ()  [unwired: 10 in]
            n155 = Select(t=Commande_1."Bras 2", s=w369, f=Commande_1."Intersection") -> (s? t:f=w372:T2)
          }
          frame "Bras 2" {
            n156 = flat-sequence {
              frame #0 {
                n157 = while {
                  i -> [w386]
                  stop <- w384 stop-if-true
                  n158 = Less?(x=1500, y=w386) -> (x < y?=w384:bool)
                  n159 = call "Sous_VI_acq_ligne.vi"("Seuil"=150) -> ("Décalage"=w383:u32, "G/D ?"=w382:bool)  [unwired: 10 in, 3 out]
                  n160 = call "Sous_VI_correction.vi"("G/D ?"=w382, "Décalage"=w383) -> ()  [unwired: 10 in]
                }
              }
              frame #1 {
                n161 = while {
                  i -> [w390]
                  stop <- w388 stop-if-true
                  w387 = 0.0 ("moteur gauche vite")
                  n162 = Less?(x=1500, y=w390) -> (x < y?=w388:bool)
                  n163 = call "Sous_VI_moteurs.vi"("Moteur Droit"=w387, "Moteur Gauche"=w387) -> ()  [unwired: 10 in]
                }
              }
              frame #2 {
                n164 = while {
                  shift-right: [w396] -> _
                  shift-left: 0 -> [w392]
                  stop <- w394 stop-if-true
                  n165 = Greater Or Equal?(x=w392, y=1500) -> (x >= y?=w395:bool)
                  n166 = case shown="False" w395 {
                    tunnel: [FALSE TRUE] -> w394
                    frame False {
                      n167 = call "Sous_VI_Bras.vi"("Enum bras"=enum_bras."Clapet Bras") -> ()  [unwired: 11 in]
                    }
                    frame True {
                    }
                  }
                  n168 = Increment(x=w392) -> (x+1=w396:i32)
                }
              }
            }
          }
          frame "Clapet 2" {
            n169 = call "Sous_VI_acq_ligne.vi"("Seuil"=150) -> ("Décalage"=w407:u32, "G/D ?"=w406:bool)  [unwired: 10 in, 3 out]
            n170 = call "Sous_VI_correction.vi"("G/D ?"=w406, "Décalage"=w407) -> ()  [unwired: 10 in]
            n171 = Select(t=Commande_1."Monter_bras2", s=w400, f=Commande_1."Clapet 2") -> (s? t:f=w402:T2)
          }
          frame "Monter_bras2" {
            n172 = call "Sous_VI_Monter_Bras.vi"() -> ()  [unwired: 12 in]
          }
          frame "Avance3" {
            n173 = call "Sous_VI_acq_ligne.vi"("Seuil"=150) -> ("Décalage"=w418:u32, "G/D ?"=w417:bool)  [unwired: 10 in, 3 out]
            n174 = call "Sous_VI_correction.vi"("G/D ?"=w417, "Décalage"=w418) -> ()  [unwired: 10 in]
            n175 = Select(t=Commande_1."Virage 3", s=w413, f=Commande_1."Avance3") -> (s? t:f=w414:T2)
          }
          frame "Virage 3" {
            n176 = call "Sous_VI_Virage_1.vi"() -> ()  [unwired: 12 in]
          }
          frame "Avance" {
            n177 = call "Sous_VI_acq_ligne.vi"("Seuil"=150) -> ("Décalage"=w427:u32, "G/D ?"=w426:bool)  [unwired: 10 in, 3 out]
            n178 = call "Sous_VI_correction.vi"("G/D ?"=w426, "Décalage"=w427) -> ()  [unwired: 10 in]
            n179 = Select(t=Commande_1."Virage 4", s=w428, f=Commande_1."Avance") -> (s? t:f=w429:T2)
          }
          frame "Virage 4" {
            n180 = call "Sous_VI_Virage_1.vi"() -> ()  [unwired: 12 in]
          }
          frame "Lanceur" {
            n181 = call "Sous_VI_Lanceur.vi"("Nb balles"=1) -> ()  [unwired: 11 in]
          }
          frame "Demi_tour" {
            n182 = call "Sous_VI_Virage_1.vi"() -> ()  [unwired: 12 in]
          }
          frame "Virage 5" {
            n183 = case shown="True" w445 {
              tunnel: [Commande_1."Virage 5" Commande_1."Virage 6"] -> w446
              frame False {
                n184 = call "Sous_VI_acq_ligne.vi"("Seuil"=150) -> ("Décalage"=w450:u32, "G/D ?"=w449:bool)  [unwired: 10 in, 3 out]
                n185 = call "Sous_VI_correction.vi"("G/D ?"=w449, "Décalage"=w450) -> ()  [unwired: 10 in]
              }
              frame True {
                n186 = call "Sous_VI_Virage_cible.vi"() -> ()  [unwired: 12 in]
              }
            }
          }
          frame "Virage 6" {
            n187 = case shown="True" w455 {
              tunnel: [Commande_1."Virage 6" Commande_1."End"] -> w454
              frame False {
                n188 = call "Sous_VI_acq_ligne.vi"("Seuil"=150) -> ("Décalage"=w459:u32, "G/D ?"=w458:bool)  [unwired: 10 in, 3 out]
                n189 = call "Sous_VI_correction.vi"("G/D ?"=w458, "Décalage"=w459) -> ()  [unwired: 10 in]
              }
              frame True {
                n190 = call "Sous_VI_Virage_1.vi"() -> ()  [unwired: 12 in]
              }
            }
          }
          frame "End" {
          }
        }
      }
      frame "Tour3" {
        n191 = case shown="\"Virage 4\"" w464 {
          tunnel: [w471 w487 Commande_1."Clapet 1" w511 Commande_1."Sceaux 0" w520 w538 w554 w569 w582 w598 w608 Commande_1."Intersection" w627 w642 Commande_1."Clapet 2" w661 Commande_1."Avance" w689 Commande_1."Lanceur" Commande_1."Demi_tour" Commande_1."Virage 5" w706 w714 Commande_1."End"] -> w469
          tunnel: w465 -> [_ _ _ w505 _ _ _ _ _ _ w597 _ _ _ _ _ w659 _ w688 _ _ _ w705 w715 _]
          tunnel: [T1 {"Bras"=TRUE, "Avance"=TRUE, "Tourne"=FALSE, "Sceaux"=FALSE, "Virage 2"=FALSE, "Trieur"=FALSE, "Bras 2"=FALSE, "Clapet 2"=FALSE, "Virage 3"=FALSE, "Virage 4"=FALSE, "Lanceur"=FALSE} ("Cluster 2") T1 {"Bras"=TRUE, "Avance"=TRUE, "Tourne"=FALSE, "Sceaux"=FALSE, "Virage 2"=FALSE, "Trieur"=FALSE, "Bras 2"=FALSE, "Clapet 2"=FALSE, "Virage 3"=FALSE, "Virage 4"=FALSE, "Lanceur"=FALSE} ("Cluster 2") T1 {"Bras"=TRUE, "Avance"=TRUE, "Tourne"=FALSE, "Sceaux"=FALSE, "Virage 2"=FALSE, "Trieur"=FALSE, "Bras 2"=FALSE, "Clapet 2"=FALSE, "Virage 3"=FALSE, "Virage 4"=FALSE, "Lanceur"=FALSE} ("Cluster 2") T1 {"Bras"=TRUE, "Avance"=TRUE, "Tourne"=TRUE, "Sceaux"=FALSE, "Virage 2"=FALSE, "Trieur"=FALSE, "Bras 2"=FALSE, "Clapet 2"=FALSE, "Virage 3"=FALSE, "Virage 4"=FALSE, "Lanceur"=FALSE} ("Cluster 2") T1 {"Bras"=TRUE, "Avance"=TRUE, "Tourne"=TRUE, "Sceaux"=TRUE, "Virage 2"=FALSE, "Trieur"=FALSE, "Bras 2"=FALSE, "Clapet 2"=FALSE, "Virage 3"=FALSE, "Virage 4"=FALSE, "Lanceur"=FALSE} ("Cluster 2") T1 {"Bras"=TRUE, "Avance"=TRUE, "Tourne"=TRUE, "Sceaux"=TRUE, "Virage 2"=TRUE, "Trieur"=TRUE, "Bras 2"=TRUE, "Clapet 2"=TRUE, "Virage 3"=TRUE, "Virage 4"=TRUE, "Lanceur"=TRUE} ("Cluster 2") w537 w553 w571 T1 {"Bras"=TRUE, "Avance"=TRUE, "Tourne"=TRUE, "Sceaux"=TRUE, "Virage 2"=TRUE, "Trieur"=TRUE, "Bras 2"=TRUE, "Clapet 2"=TRUE, "Virage 3"=TRUE, "Virage 4"=TRUE, "Lanceur"=TRUE} ("Cluster 2") w601 T1 {"Bras"=TRUE, "Avance"=TRUE, "Tourne"=TRUE, "Sceaux"=TRUE, "Virage 2"=TRUE, "Trieur"=FALSE, "Bras 2"=FALSE, "Clapet 2"=FALSE, "Virage 3"=FALSE, "Virage 4"=FALSE, "Lanceur"=FALSE} ("Cluster 2") T1 {"Bras"=FALSE, "Avance"=FALSE, "Tourne"=FALSE, "Sceaux"=FALSE, "Virage 2"=FALSE, "Trieur"=FALSE, "Bras 2"=FALSE, "Clapet 2"=FALSE, "Virage 3"=FALSE, "Virage 4"=FALSE, "Lanceur"=FALSE} ("Cluster 2") T1 {"Bras"=FALSE, "Avance"=FALSE, "Tourne"=FALSE, "Sceaux"=FALSE, "Virage 2"=FALSE, "Trieur"=TRUE, "Bras 2"=TRUE, "Clapet 2"=FALSE, "Virage 3"=FALSE, "Virage 4"=FALSE, "Lanceur"=FALSE} ("Cluster 2") T1 {"Bras"=FALSE, "Avance"=FALSE, "Tourne"=FALSE, "Sceaux"=FALSE, "Virage 2"=FALSE, "Trieur"=TRUE, "Bras 2"=TRUE, "Clapet 2"=FALSE, "Virage 3"=FALSE, "Virage 4"=FALSE, "Lanceur"=FALSE} ("Cluster 2") T1 {"Bras"=FALSE, "Avance"=FALSE, "Tourne"=FALSE, "Sceaux"=FALSE, "Virage 2"=FALSE, "Trieur"=TRUE, "Bras 2"=FALSE, "Clapet 2"=FALSE, "Virage 3"=FALSE, "Virage 4"=FALSE, "Lanceur"=FALSE} ("Cluster 2") T1 {"Bras"=FALSE, "Avance"=FALSE, "Tourne"=FALSE, "Sceaux"=FALSE, "Virage 2"=FALSE, "Trieur"=TRUE, "Bras 2"=TRUE, "Clapet 2"=FALSE, "Virage 3"=FALSE, "Virage 4"=FALSE, "Lanceur"=FALSE} ("Cluster 2") T1 {"Bras"=FALSE, "Avance"=FALSE, "Tourne"=FALSE, "Sceaux"=FALSE, "Virage 2"=FALSE, "Trieur"=TRUE, "Bras 2"=TRUE, "Clapet 2"=TRUE, "Virage 3"=TRUE, "Virage 4"=FALSE, "Lanceur"=FALSE} ("Cluster 2") T1 {"Bras"=FALSE, "Avance"=FALSE, "Tourne"=FALSE, "Sceaux"=FALSE, "Virage 2"=FALSE, "Trieur"=FALSE, "Bras 2"=TRUE, "Clapet 2"=TRUE, "Virage 3"=TRUE, "Virage 4"=TRUE, "Lanceur"=FALSE} ("Cluster 2") T1 {"Bras"=FALSE, "Avance"=FALSE, "Tourne"=FALSE, "Sceaux"=FALSE, "Virage 2"=FALSE, "Trieur"=TRUE, "Bras 2"=TRUE, "Clapet 2"=TRUE, "Virage 3"=TRUE, "Virage 4"=TRUE, "Lanceur"=FALSE} ("Cluster 2") T1 {"Bras"=FALSE, "Avance"=FALSE, "Tourne"=FALSE, "Sceaux"=FALSE, "Virage 2"=FALSE, "Trieur"=FALSE, "Bras 2"=TRUE, "Clapet 2"=TRUE, "Virage 3"=TRUE, "Virage 4"=TRUE, "Lanceur"=TRUE} ("Cluster 2") T1 {"Bras"=FALSE, "Avance"=FALSE, "Tourne"=FALSE, "Sceaux"=FALSE, "Virage 2"=FALSE, "Trieur"=TRUE, "Bras 2"=TRUE, "Clapet 2"=TRUE, "Virage 3"=TRUE, "Virage 4"=TRUE, "Lanceur"=FALSE} ("Cluster 2") T1 {"Bras"=FALSE, "Avance"=FALSE, "Tourne"=FALSE, "Sceaux"=FALSE, "Virage 2"=FALSE, "Trieur"=TRUE, "Bras 2"=TRUE, "Clapet 2"=TRUE, "Virage 3"=TRUE, "Virage 4"=TRUE, "Lanceur"=FALSE} ("Cluster 2") T1 {"Bras"=FALSE, "Avance"=FALSE, "Tourne"=FALSE, "Sceaux"=FALSE, "Virage 2"=FALSE, "Trieur"=TRUE, "Bras 2"=TRUE, "Clapet 2"=TRUE, "Virage 3"=TRUE, "Virage 4"=TRUE, "Lanceur"=FALSE} ("Cluster 2") T1 {"Bras"=FALSE, "Avance"=FALSE, "Tourne"=FALSE, "Sceaux"=FALSE, "Virage 2"=FALSE, "Trieur"=FALSE, "Bras 2"=FALSE, "Clapet 2"=FALSE, "Virage 3"=FALSE, "Virage 4"=FALSE, "Lanceur"=FALSE} ("Cluster 2")] -> w468
          tunnel: w466 -> [w470 w488 _ _ _ w519 w536 w555 w572 _ _ w609 _ w624 w643 _ _ _ _ _ _ _ _ _ _]
          tunnel: [enum_tour."Tour3" enum_tour."Tour3" enum_tour."Tour3" enum_tour."Tour3" enum_tour."Tour3" enum_tour."Tour3" enum_tour."Tour3" enum_tour."Tour3" enum_tour."Tour3" enum_tour."Tour3" enum_tour."Tour3" enum_tour."Tour3" enum_tour."Tour3" enum_tour."Tour3" enum_tour."Tour3" enum_tour."Tour3" enum_tour."Tour3" enum_tour."Tour3" enum_tour."Tour3" enum_tour."Tour3" enum_tour."Tour3" enum_tour."Tour3" enum_tour."Tour3" enum_tour."Tour3" enum_tour."Tour3"] -> w467
          frame "Intersection2", Default {
            n192 = Select(t=Commande_1."Intersection3", s=w470, f=Commande_1."Intersection2") -> (s? t:f=w471:T2)
            n193 = case shown="True" w470 {
              frame False {
                n194 = call "Sous_VI_acq_ligne.vi"("Seuil"=150) -> ("Décalage"=w476:u32, "G/D ?"=w477:bool)  [unwired: 10 in, 3 out]
                n195 = call "Sous_VI_correction.vi"("G/D ?"=w477, "Décalage"=w476) -> ()  [unwired: 10 in]
              }
              frame True {
                n196 = while {
                  i -> [w484]
                  stop <- w479 stop-if-true
                  n197 = call "Sous_VI_acq_ligne.vi"("Seuil"=150) -> ("Décalage"=w480:u32, "G/D ?"=w481:bool)  [unwired: 10 in, 3 out]
                  n198 = call "Sous_VI_correction.vi"("G/D ?"=w481, "Décalage"=w480) -> ()  [unwired: 10 in]
                  n199 = Greater Or Equal?(x=w484, y=200) -> (x >= y?=w479:bool)
                }
              }
            }
          }
          frame "Intersection3" {
            n200 = call "Sous_VI_acq_ligne.vi"("Seuil"=150) -> ("Décalage"=w491:u32, "G/D ?"=w490:bool)  [unwired: 10 in, 3 out]
            n201 = call "Sous_VI_correction.vi"("G/D ?"=w490, "Décalage"=w491) -> ()  [unwired: 10 in]
            n202 = Select(t=Commande_1."Bras", s=w488, f=Commande_1."Intersection3") -> (s? t:f=w487:T2)
          }
          frame "Bras" {
            n203 = flat-sequence {
              frame #0 {
                n204 = while {
                  i -> [w502]
                  stop <- w500 stop-if-true
                  n205 = Less?(x=1500, y=w502) -> (x < y?=w500:bool)
                  n206 = call "Sous_VI_acq_ligne.vi"("Seuil"=150) -> ("Décalage"=w498:u32, "G/D ?"=w497:bool)  [unwired: 10 in, 3 out]
                  n207 = call "Sous_VI_correction.vi"("G/D ?"=w497, "Décalage"=w498) -> ()  [unwired: 10 in]
                }
              }
              frame #1 {
                w503 = 0.0 ("moteur gauche vite")
                n208 = call "Sous_VI_moteurs.vi"("Moteur Droit"=w503, "Moteur Gauche"=w503) -> ()  [unwired: 10 in]
              }
              frame #2 {
                n209 = call "Sous_VI_Bras.vi"("Enum bras"=enum_bras."Clapet Bras") -> ()  [unwired: 11 in]
              }
            }
          }
          frame "Clapet 1" {
            n210 = call "Sous_VI_acq_ligne.vi"("Seuil"=150) -> ("Décalage"=w509:u32, "G/D ?"=w508:bool)  [unwired: 10 in, 3 out]
            n211 = Select(t=Commande_1."Virage 1", s=w505, f=Commande_1."Clapet 1") -> (s? t:f=w511:T2)
            n212 = call "Sous_VI_correction.vi"("G/D ?"=w508, "Décalage"=w509) -> ()  [unwired: 10 in]
          }
          frame "Virage 1" {
            n213 = call "Sous_VI_Virage_1.vi"() -> ()  [unwired: 12 in]
          }
          frame "Sceaux 0" {
            n214 = case shown="True" w519 {
              tunnel: [Commande_1."Sceaux 0" Commande_1."Sceaux 1"] -> w520
              frame False {
                n215 = call "Sous_VI_acq_ligne.vi"("Seuil"=150) -> ("Décalage"=w523:u32, "G/D ?"=w522:bool)  [unwired: 10 in, 3 out]
                n216 = call "Sous_VI_correction.vi"("G/D ?"=w522, "Décalage"=w523) -> ()  [unwired: 10 in]
              }
              frame True {
                n217 = while {
                  i -> [w529]
                  stop <- w526 stop-if-true
                  n218 = Greater Or Equal?(x=w529, y=200) -> (x >= y?=w527:bool)
                  n219 = case shown="False" w527 {
                    tunnel: [FALSE TRUE] -> w526
                    frame False {
                      n220 = call "Sous_VI_acq_ligne.vi"("Seuil"=150) -> ("Décalage"=w533:u32, "G/D ?"=w532:bool)  [unwired: 10 in, 3 out]
                      n221 = call "Sous_VI_correction.vi"("G/D ?"=w532, "Décalage"=w533) -> ()  [unwired: 10 in]
                    }
                    frame True {
                    }
                  }
                }
              }
            }
          }
          frame "Sceaux 1" {
            n222 = Select(t=Commande_1."Sceaux 2", s=w536, f=Commande_1."Sceaux 1") -> (s? t:f=w538:T2)
            n223 = case shown="True" w536 {
              tunnel: [T1 {"Bras"=TRUE, "Avance"=TRUE, "Tourne"=TRUE, "Sceaux"=FALSE, "Virage 2"=FALSE, "Trieur"=FALSE, "Bras 2"=FALSE, "Clapet 2"=FALSE, "Virage 3"=FALSE, "Virage 4"=FALSE, "Lanceur"=FALSE} ("Cluster 2") T1 {"Bras"=TRUE, "Avance"=TRUE, "Tourne"=TRUE, "Sceaux"=TRUE, "Virage 2"=TRUE, "Trieur"=TRUE, "Bras 2"=TRUE, "Clapet 2"=TRUE, "Virage 3"=TRUE, "Virage 4"=TRUE, "Lanceur"=TRUE} ("Cluster 2")] -> w537
              frame False {
                n224 = call "Sous_VI_acq_ligne.vi"("Seuil"=150) -> ("Décalage"=w543:u32, "G/D ?"=w542:bool)  [unwired: 10 in, 3 out]
                n225 = call "Sous_VI_correction.vi"("G/D ?"=w542, "Décalage"=w543) -> ()  [unwired: 10 in]
              }
              frame True {
                n226 = while {
                  i -> [w551]
                  stop <- w546 stop-if-true
                  n227 = call "Sous_VI_acq_ligne.vi"("Seuil"=150) -> ("Décalage"=w547:u32, "G/D ?"=w548:bool)  [unwired: 10 in, 3 out]
                  n228 = call "Sous_VI_correction.vi"("G/D ?"=w548, "Décalage"=w547) -> ()  [unwired: 10 in]
                  n229 = Greater Or Equal?(x=w551, y=200) -> (x >= y?=w546:bool)
                }
              }
            }
          }
          frame "Sceaux 2" {
            n230 = Select(t=Commande_1."Sceaux 3", s=w555, f=Commande_1."Sceaux 2") -> (s? t:f=w554:T2)
            n231 = case shown="True" w555 {
              tunnel: [T1 {"Bras"=TRUE, "Avance"=TRUE, "Tourne"=TRUE, "Sceaux"=FALSE, "Virage 2"=FALSE, "Trieur"=FALSE, "Bras 2"=FALSE, "Clapet 2"=FALSE, "Virage 3"=FALSE, "Virage 4"=FALSE, "Lanceur"=FALSE} ("Cluster 2") T1 {"Bras"=TRUE, "Avance"=TRUE, "Tourne"=TRUE, "Sceaux"=TRUE, "Virage 2"=TRUE, "Trieur"=TRUE, "Bras 2"=TRUE, "Clapet 2"=TRUE, "Virage 3"=TRUE, "Virage 4"=TRUE, "Lanceur"=TRUE} ("Cluster 2")] -> w553
              frame False {
                n232 = call "Sous_VI_acq_ligne.vi"("Seuil"=150) -> ("Décalage"=w560:u32, "G/D ?"=w559:bool)  [unwired: 10 in, 3 out]
                n233 = call "Sous_VI_correction.vi"("G/D ?"=w559, "Décalage"=w560) -> ()  [unwired: 10 in]
              }
              frame True {
                n234 = while {
                  i -> [w568]
                  stop <- w563 stop-if-true
                  n235 = call "Sous_VI_acq_ligne.vi"("Seuil"=150) -> ("Décalage"=w564:u32, "G/D ?"=w565:bool)  [unwired: 10 in, 3 out]
                  n236 = call "Sous_VI_correction.vi"("G/D ?"=w565, "Décalage"=w564) -> ()  [unwired: 10 in]
                  n237 = Greater Or Equal?(x=w568, y=200) -> (x >= y?=w563:bool)
                }
              }
            }
          }
          frame "Sceaux 3" {
            n238 = Select(t=Commande_1."Sceaux 4", s=w572, f=Commande_1."Sceaux 3") -> (s? t:f=w569:T2)
            n239 = case shown="True" w572 {
              tunnel: [T1 {"Bras"=TRUE, "Avance"=TRUE, "Tourne"=TRUE, "Sceaux"=FALSE, "Virage 2"=FALSE, "Trieur"=FALSE, "Bras 2"=FALSE, "Clapet 2"=FALSE, "Virage 3"=FALSE, "Virage 4"=FALSE, "Lanceur"=FALSE} ("Cluster 2") T1 {"Bras"=TRUE, "Avance"=TRUE, "Tourne"=TRUE, "Sceaux"=TRUE, "Virage 2"=TRUE, "Trieur"=TRUE, "Bras 2"=TRUE, "Clapet 2"=TRUE, "Virage 3"=TRUE, "Virage 4"=TRUE, "Lanceur"=TRUE} ("Cluster 2")] -> w571
              frame False {
                n240 = call "Sous_VI_acq_ligne.vi"("Seuil"=150) -> ("Décalage"=w577:u32, "G/D ?"=w576:bool)  [unwired: 10 in, 3 out]
                n241 = call "Sous_VI_correction.vi"("G/D ?"=w576, "Décalage"=w577) -> ()  [unwired: 10 in]
              }
              frame True {
                n242 = call "Sous_VI_Sceaux.vi"() -> ()  [unwired: 12 in]
              }
            }
          }
          frame "Sceaux 4" {
            n243 = flat-sequence {
              tunnel: [Commande_1."Virage 2"] -> w582
              frame #0 {
                n244 = while {
                  i -> [w586]
                  stop <- w583 stop-if-true
                  n245 = Greater Or Equal?(x=w586, y=400) -> (x >= y?=w584:bool)
                  n246 = case shown="False" w584 {
                    tunnel: [FALSE TRUE] -> w583
                    frame False {
                      n247 = call "Sous_VI_acq_ligne.vi"("Seuil"=150) -> ("Décalage"=w589:u32, "G/D ?"=w588:bool)  [unwired: 10 in, 3 out]
                      n248 = call "Sous_VI_correction.vi"("G/D ?"=w588, "Décalage"=w589) -> ()  [unwired: 10 in]
                    }
                    frame True {
                    }
                  }
                }
              }
              frame #1 {
                n249 = call "Sous_VI_Sceaux.vi"() -> ()  [unwired: 12 in]
              }
              frame #2 {
                n250 = call "Sous_VI_acq_ligne.vi"("Seuil"=150) -> ("Décalage"=w595:u32, "G/D ?"=w594:bool)  [unwired: 10 in, 3 out]
                n251 = call "Sous_VI_correction.vi"("G/D ?"=w594, "Décalage"=w595) -> ()  [unwired: 10 in]
              }
            }
          }
          frame "Virage 2" {
            n252 = Select(t=Commande_1."Recule", s=w597, f=Commande_1."Virage 2") -> (s? t:f=w598:T2)
            n253 = case shown="True" w597 {
              tunnel: [T1 {"Bras"=TRUE, "Avance"=TRUE, "Tourne"=TRUE, "Sceaux"=FALSE, "Virage 2"=FALSE, "Trieur"=FALSE, "Bras 2"=FALSE, "Clapet 2"=FALSE, "Virage 3"=FALSE, "Virage 4"=FALSE, "Lanceur"=FALSE} ("Cluster 2") T1 {"Bras"=TRUE, "Avance"=TRUE, "Tourne"=TRUE, "Sceaux"=TRUE, "Virage 2"=FALSE, "Trieur"=FALSE, "Bras 2"=FALSE, "Clapet 2"=FALSE, "Virage 3"=FALSE, "Virage 4"=FALSE, "Lanceur"=FALSE} ("Cluster 2")] -> w601
              frame False {
                n254 = call "Sous_VI_acq_ligne.vi"("Seuil"=150) -> ("Décalage"=w604:u32, "G/D ?"=w603:bool)  [unwired: 10 in, 3 out]
                n255 = call "Sous_VI_correction.vi"("G/D ?"=w603, "Décalage"=w604) -> ()  [unwired: 10 in]
              }
              frame True {
                n256 = call "Sous_VI_Virage_1.vi"() -> ()  [unwired: 12 in]
              }
            }
          }
          frame "Recule" {
            n257 = case shown="True" w609 {
              tunnel: [Commande_1."Recule" Commande_1."Trieur"] -> w608
              frame False {
                n258 = call "Sous_VI_acq_ligne.vi"("Seuil"=150) -> ("Décalage"=w611:u32, "G/D ?"=w614:bool)  [unwired: 10 in, 3 out]
                n259 = call "Sous_VI_correction.vi"("G/D ?"=w614, "Décalage"=w611) -> ()  [unwired: 10 in]
              }
              frame True {
                n260 = call "Sous_VI_recule.vi"() -> ()  [unwired: 12 in]
              }
            }
          }
          frame "Trieur" {
            n261 = flat-sequence {
              frame #0 {
                n262 = while {
                  i -> [w621]
                  stop <- w619 stop-if-true
                  w622 = 0.0 ("moteur gauche vite")
                  n263 = Less?(x=2000, y=w621) -> (x < y?=w619:bool)
                  n264 = call "Sous_VI_moteurs.vi"("Moteur Droit"=w622, "Moteur Gauche"=w622) -> ()  [unwired: 10 in]
                }
              }
              frame #1 {
                n265 = call "Labview_trieur_balles.vi"("Numeric"=4) -> ()  [unwired: 11 in]
              }
            }
          }
          frame "Intersection" {
            n266 = Select(t=Commande_1."Intersection4", s=w624, f=Commande_1."Intersection") -> (s? t:f=w627:T2)
            n267 = case shown="True" w624 {
              frame False {
                n268 = call "Sous_VI_acq_ligne.vi"("Seuil"=150) -> ("Décalage"=w630:u32, "G/D ?"=w631:bool)  [unwired: 10 in, 3 out]
                n269 = call "Sous_VI_correction.vi"("G/D ?"=w631, "Décalage"=w630) -> ()  [unwired: 10 in]
              }
              frame True {
                n270 = while {
                  i -> [w638]
                  stop <- w633 stop-if-true
                  n271 = call "Sous_VI_acq_ligne.vi"("Seuil"=150) -> ("Décalage"=w634:u32, "G/D ?"=w635:bool)  [unwired: 10 in, 3 out]
                  n272 = call "Sous_VI_correction.vi"("G/D ?"=w635, "Décalage"=w634) -> ()  [unwired: 10 in]
                  n273 = Greater Or Equal?(x=w638, y=200) -> (x >= y?=w633:bool)
                }
              }
            }
          }
          frame "Intersection4" {
            n274 = call "Sous_VI_acq_ligne.vi"("Seuil"=150) -> ("Décalage"=w639:u32, "G/D ?"=w647:bool)  [unwired: 10 in, 3 out]
            n275 = call "Sous_VI_correction.vi"("G/D ?"=w647, "Décalage"=w639) -> ()  [unwired: 10 in]
            n276 = Select(t=Commande_1."Bras 2", s=w643, f=Commande_1."Intersection4") -> (s? t:f=w642:T2)
          }
          frame "Bras 2" {
            n277 = flat-sequence {
              frame #0 {
                n278 = while {
                  i -> [w656]
                  stop <- w654 stop-if-true
                  n279 = Less?(x=1500, y=w656) -> (x < y?=w654:bool)
                  n280 = call "Sous_VI_acq_ligne.vi"("Seuil"=150) -> ("Décalage"=w652:u32, "G/D ?"=w651:bool)  [unwired: 10 in, 3 out]
                  n281 = call "Sous_VI_correction.vi"("G/D ?"=w651, "Décalage"=w652) -> ()  [unwired: 10 in]
                }
              }
              frame #1 {
                w657 = 0.0 ("moteur gauche vite")
                n282 = call "Sous_VI_moteurs.vi"("Moteur Droit"=w657, "Moteur Gauche"=w657) -> ()  [unwired: 10 in]
              }
              frame #2 {
                n283 = call "Sous_VI_Bras.vi"("Enum bras"=enum_bras."Clapet Bras") -> ()  [unwired: 11 in]
              }
            }
          }
          frame "Clapet 2" {
            n284 = call "Sous_VI_acq_ligne.vi"("Seuil"=150) -> ("Décalage"=w666:u32, "G/D ?"=w665:bool)  [unwired: 10 in, 3 out]
            n285 = call "Sous_VI_correction.vi"("G/D ?"=w665, "Décalage"=w666) -> ()  [unwired: 10 in]
            n286 = Select(t=Commande_1."Virage 3", s=w659, f=Commande_1."Clapet 2") -> (s? t:f=w661:T2)
          }
          frame "Virage 3" {
            n287 = flat-sequence {
              frame #0 {
                n288 = while {
                  i -> [w672]
                  stop <- w671 stop-if-true
                  w674 = 0.0 ("moteur gauche vite")
                  n289 = call "Sous_VI_moteurs.vi"("Moteur Droit"=w674, "Moteur Gauche"=w674) -> ()  [unwired: 10 in]
                  n290 = Less?(x=1000, y=w672) -> (x < y?=w671:bool)
                }
              }
              frame #1 {
                n291 = while {
                  shift-right: [w680] -> _
                  shift-left: 0 -> [w676]
                  stop <- w678 stop-if-true
                  n292 = Greater Or Equal?(x=w676, y=100000) -> (x >= y?=w679:bool)
                  n293 = case shown="False" w679 {
                    tunnel: [FALSE TRUE] -> w678
                    frame False {
                      n294 = call "Sous_VI_Bras.vi"("Enum bras"=enum_bras."Inactif Bras") -> ()  [unwired: 11 in]
                    }
                    frame True {
                    }
                  }
                  n295 = Increment(x=w676) -> (x+1=w680:i32)
                }
              }
              frame #2 {
                n296 = call "Sous_VI_Virage_1.vi"() -> ()  [unwired: 12 in]
              }
            }
          }
          frame "Avance" {
            n297 = call "Sous_VI_acq_ligne.vi"("Seuil"=150) -> ("Décalage"=w687:u32, "G/D ?"=w686:bool)  [unwired: 10 in, 3 out]
            n298 = call "Sous_VI_correction.vi"("G/D ?"=w686, "Décalage"=w687) -> ()  [unwired: 10 in]
            n299 = Select(t=Commande_1."Virage 4", s=w688, f=Commande_1."Avance") -> (s? t:f=w689:T2)
          }
          frame "Virage 4" {
            n300 = call "Sous_VI_Virage_1.vi"() -> ()  [unwired: 12 in]
          }
          frame "Lanceur" {
            n301 = call "Sous_VI_Lanceur.vi"("Nb balles"=2) -> ()  [unwired: 11 in]
          }
          frame "Demi_tour" {
            n302 = call "Sous_VI_Virage_1.vi"() -> ()  [unwired: 12 in]
          }
          frame "Virage 5" {
            n303 = case shown="True" w705 {
              tunnel: [Commande_1."Virage 5" Commande_1."Virage 6"] -> w706
              frame False {
                n304 = call "Sous_VI_acq_ligne.vi"("Seuil"=150) -> ("Décalage"=w710:u32, "G/D ?"=w709:bool)  [unwired: 10 in, 3 out]
                n305 = call "Sous_VI_correction.vi"("G/D ?"=w709, "Décalage"=w710) -> ()  [unwired: 10 in]
              }
              frame True {
                n306 = call "Sous_VI_Virage_cible.vi"() -> ()  [unwired: 12 in]
              }
            }
          }
          frame "Virage 6" {
            n307 = case shown="True" w715 {
              tunnel: [Commande_1."Virage 6" Commande_1."End"] -> w714
              frame False {
                n308 = call "Sous_VI_acq_ligne.vi"("Seuil"=150) -> ("Décalage"=w719:u32, "G/D ?"=w718:bool)  [unwired: 10 in, 3 out]
                n309 = call "Sous_VI_correction.vi"("G/D ?"=w718, "Décalage"=w719) -> ()  [unwired: 10 in]
              }
              frame True {
                n310 = call "Sous_VI_Virage_1.vi"() -> ()  [unwired: 12 in]
              }
            }
          }
          frame "End" {
            w721 = 0.0 ("moteur gauche vite")
            n311 = call "Sous_VI_moteurs.vi"("Moteur Droit"=w721, "Moteur Gauche"=w721) -> ()  [unwired: 10 in]
          }
        }
      }
    }
    "Cluster 3" <- w23
    "Énum 2" <- w29
    n312 = node-c288() -> ()  [unwired: 1 in, 1 out]
  }
  n313 = node-c288(w5) -> ()  [unwired: 1 out]
